vi "Machine_Etat_M1.vi"() -> ()   [LabVIEW 2017]
uses:
  Commande 1.ctl
  enum_tour.ctl
  <vilib>/Platform/TimedLoop/XDataNode/timing_clust.ctl
  <vilib>/Platform/TimedLoop/XDataNode/nitl_modes.ctl
  <vilib>/Platform/TimedLoop/XDataNode/wakeup.ctl
  <vilib>/myRIO/Instrument Drivers/Onboard IO/DIO/typedefs/DIO Reference.ctl
  <vilib>/myRIO/Common/Instrument Driver Framework/Utilities/typedefs/myRIO Generic Hardware Reference.ctl
  <vilib>/myRIO/Common/Instrument Driver Framework/Utilities/typedefs/Hardware Version Enum.ctl
  <vilib>/myRIO/Common/Instrument Driver Framework/Utilities/typedefs/myRIO v1.0 Reference.ctl
  <vilib>/myRIO/Common/Instrument Driver Framework/Utilities/typedefs/Generic FPGA Reference.ctl
  <vilib>/myRIO/Common/Instrument Driver Framework/myRIO v1.0/DIO/typedefs/DIO Channels List.ctl
  <vilib>/myRIO/Common/Instrument Driver Framework/myRIO v1.0/DIO/typedefs/DIO Channels Enum.ctl
  <vilib>/userdefined/High Color/nirio_resource_hc.ctl
  enum_bras.ctl
  <vilib>/myRIO/Common/Instrument Driver Framework/Utilities/vis/Is FPGA Ref Available.vi
  <vilib>/myRIO/Common/Instrument Driver Framework/myRIO v1.0/DIO/vis/myRIO v1.1 Open DIO.vi
  <vilib>/myRIO/Instrument Drivers/Onboard IO/DIO/vis/Write.vi
  <vilib>/myRIO/Common/Instrument Driver Framework/Utilities/vis/Validate Channels.vi
  <vilib>/myRIO/Common/Instrument Driver Framework/myRIO v1.0/DIO/vis/myRIO v1.0 Reserve DIO.vi
  <vilib>/myRIO/Common/Instrument Driver Framework/myRIO v1.0/Resource Manager/vis/myRIO v1.0 Reserve Channel List.vi
  <vilib>/myRIO/Common/Instrument Driver Framework/myRIO v1.0/DIO/vis/myRIO v1.0 Build MUX Configuration DIO.vi
  <vilib>/myRIO/Common/Instrument Driver Framework/myRIO v1.0/Resource Manager/vis/myRIO v1.0 Reserve Channel.vi
  <vilib>/myRIO/Common/Instrument Driver Framework/myRIO v1.0/Resource Manager/vis/myRIO v1.0 Unreserve Channel.vi
  <vilib>/myRIO/Common/Instrument Driver Framework/myRIO v1.0/Resource Manager/vis/myRIO v1.0 Create Configuration List.vi
  <vilib>/myRIO/Common/Instrument Driver Framework/myRIO v1.0/Resource Manager/vis/myRIO v1.0 Build Mutex Name.vi
  <vilib>/Utility/VariantDataType/GetNumericInfo.vi
  <vilib>/Utility/error.llb/Error Cluster From Error Code.vi
  <vilib>/myRIO/Common/Instrument Driver Framework/myRIO v1.0/myRIO v1.1 Open.vi
  <vilib>/myRIO/Common/Instrument Driver Framework/Utilities/vis/IO Manager.vi
  <vilib>/myRIO/Common/Instrument Driver Framework/Utilities/vis/Configuration Manager.vi
  <vilib>/myRIO/Common/Instrument Driver Framework/myRIO v1.0/Resource Manager/vis/myRIO v1.0 Configure IO.vi
  <vilib>/myRIO/Common/Instrument Driver Framework/myRIO v1.0/myRIO v1.0 Close.vi
  <vilib>/myRIO/Common/Instrument Driver Framework/myRIO v1.0/DIO/vis/myRIO v1.0 Write DIO.vi
  <vilib>/platform/TimedLoop/XDataNode/XDataNode.xnode
  <vilib>/myRIO/Express VI/Onboard Devices/LED/LED Express VI.xnode
  <vilib>/myRIO/Instrument Drivers/Onboard IO/DIO/vis/myRIO DIO Open.xnode
  <vilib>/Platform/TimedLoop/XDataNode/XDNodeRunTimeDep.lvlib
  <vilib>/myRIO/Instrument Drivers/Onboard IO/DIO/DIO.lvlib
panel:
  out "error out":errorcluster
  out "Vert : dévi à droite 2":bool
  out "Graphe déroulant 2":u32(graph)
  out "x > y ? 2":bool[](array[boolean])
  out "Cluster 3":T1
  out "4 LED droite 2":bool[](array[boolean])
  out "4 LED gauche 2":bool[](array[boolean])
  out "droite 2":u32
  out "gauche 2":u32
  out "Énum 2":T2
  out "seuil":u32
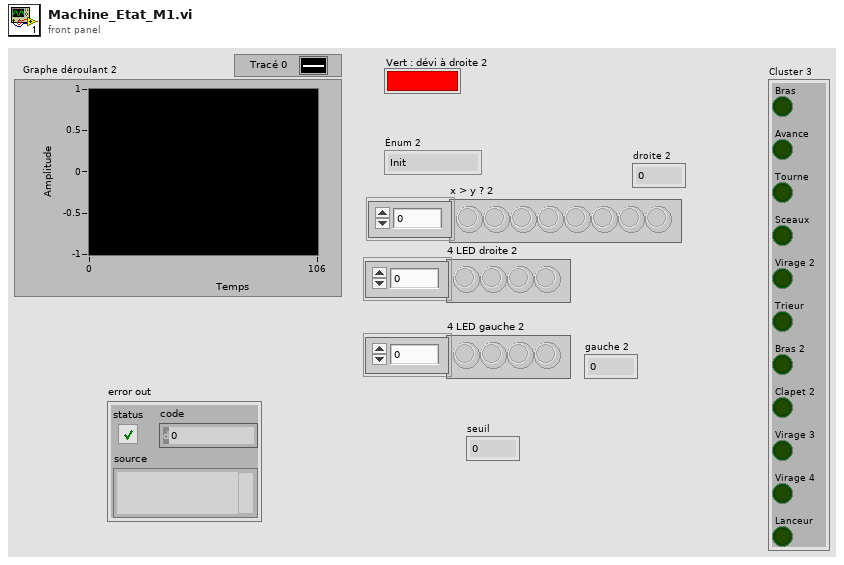
[diagram p1: front panel]
types:
  T1 = typedef "Voyant machine d'état.ctl" = cluster{"Bras":bool, "Avance":bool, "Tourne":bool, "Sceaux":bool, "Virage 2":bool, "Trieur":bool, "Bras 2":bool, "Clapet 2":bool, "Virage 3":bool, "Virage 4":bool, "Lanceur":bool}
  T2 = typedef "Commande 1.ctl" = enum16{"Init", "Bras", "Clapet 1", "Monter_bras", "Virage 1", "Sceaux 0", "Sceaux 1", "Sceaux 2", "Sceaux 3", "Sceaux 4", "Virage 2", "Recule", "Trieur", "Bras 2", "Intersection", "Clapet 2", "Virage 3", "Virage 4", "Avance", "Lanceur", "End", "Monter_bras1", "Monter_bras2", "Avance1", "Avance2", "Intersection1", "Avance3", "Demi_tour", "Virage 5", "Virage 6", "Intersection2", "Intersection3", "Intersection4"}
  T3 = typedef "enum_tour.ctl" = enum16{"Tour1", "Tour2", "Tour3"}
  T4 = typedef "XDNodeRunTimeDep.lvlib/timing_clust.ctl" = cluster{"Expected End [f-1]":u64, "Actual End [f-1]":u64, "Finished Late? [f-1]":bool, "Expected End [i-1]":u64, "Actual End [i-1]":u64, "Finished Late? [i-1]":bool, "Expected Start [i]":u64, "Actual Start [i]":u64, "Expected Start [f]":u64, "Actual Start [f]":u64, "Source Name":string, "Structure Name":string, "Period":i64, "Deadline":i64, "Offset":i64, "Start":i64, "Priority":i32, "Timeout":i32, "Mode":T5, "Wakeup Reason":T6, "Error":errorcluster, "Source Type":string, "Secondary Source Type":string, "Global End Time":u64, "Global Start Time":u64, "Frame Duration":u64, "Iteration Duration":u64, "Assigned CPU":i32, "I/O Scan Engine Mode":u32}
  T5 = typedef "XDNodeRunTimeDep.lvlib/nitl_modes.ctl" = enum32{"No Change", "Process missed periods, maintain original phase", "Discard missed periods, maintain original phase", "Process missed periods, ignore original phase", "Discard missed periods, ignore original phase"}
  T6 = typedef "XDNodeRunTimeDep.lvlib/wakeup.ctl" = enum32{"Normal", "Aborted", "Asynchronous wakeup", "Timing source error", "Timed loop error", "Timeout"}
  T7 = typedef "enum_bras.ctl" = enum16{"Depart Bras", "Clapet Bras", "Inactif Bras", "Seaux Bras"}
  T8 = typedef "DIO.lvlib/DIO Reference.ctl" = cluster{"myRIO Reference":T9, "DIO Channels List":T13}
  T9 = typedef "myRIO Generic Hardware Reference.ctl" = cluster{"myRIO Model":T10, "myRIO Hardware Reference":T11}
  T10 = typedef "Hardware Version Enum.ctl" = enum16{"Unknown", "myRIO-1900", "myRIO-1950", "roboRIO", "NI ELVIS RIO CM"}
  T11 = typedef "myRIO v1.0 Reference.ctl" = cluster{"Generic FPGA Reference":T12, "Allow multiple opens":bool}
  T12 = typedef "Generic FPGA Reference.ctl" = refnum<k20>
  T13 = typedef "DIO Channels List.ctl" = T14[]
  T14 = typedef "DIO Channels Enum.ctl" = enum16{"Not Connected", "C/DIO0", "C/DIO1", "C/DIO2", "C/DIO3", "C/DIO4", "C/DIO5", "C/DIO6", "C/DIO7", "A/DIO0", "A/DIO1", "A/DIO2", "A/DIO3", "A/DIO4", "A/DIO5", "A/DIO6", "A/DIO7", "A/DIO8", "A/DIO9", "A/DIO10", "A/DIO11", "A/DIO12", "A/DIO13", "A/DIO14", "A/DIO15", "B/DIO0", "B/DIO1", "B/DIO2", "B/DIO3", "B/DIO4", "B/DIO5", "B/DIO6", "B/DIO7", "B/DIO8", "B/DIO9", "B/DIO10", "B/DIO11", "B/DIO12", "B/DIO13", "B/DIO14", "B/DIO15", "LED0", "LED1", "LED2", "LED3", "Button0", "DIO/DIO0", "DIO/DIO1", "DIO/DIO2", "DIO/DIO3", "DIO/DIO4", "DIO/DIO5", "DIO/DIO6", "DIO/DIO7", "DIO/DIO8", "DIO/DIO9", "SPI/CS0", "SPI/CS1", "SPI/CS2", "SPI/CS3", "LED RADIO (Green)", "LED RADIO (Red)", "LED COMM (Green)", "LED COMM (Red)", "LED MODE (Green)", "LED MODE (Red)"}
  T15 = typedef "nirio_resource_hc.ctl" = tag
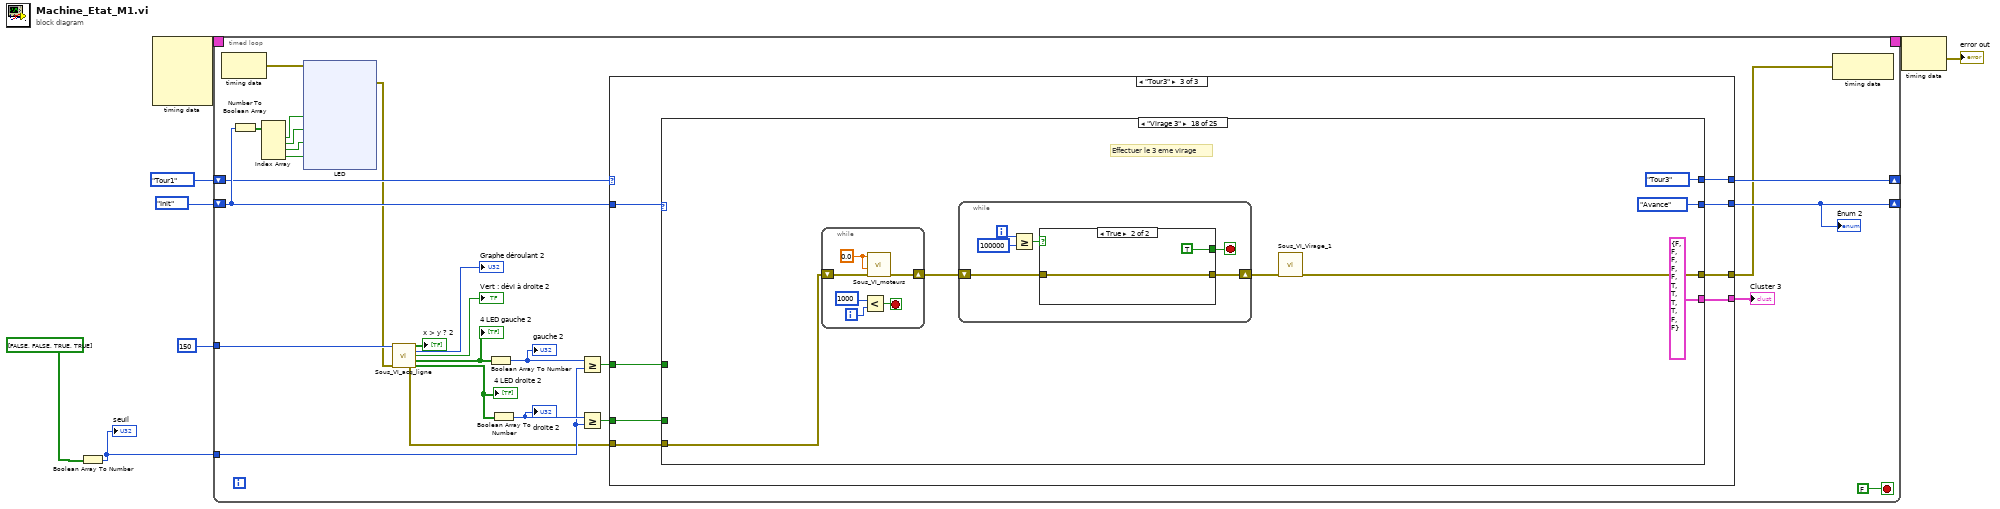
[diagram p0: block diagram]
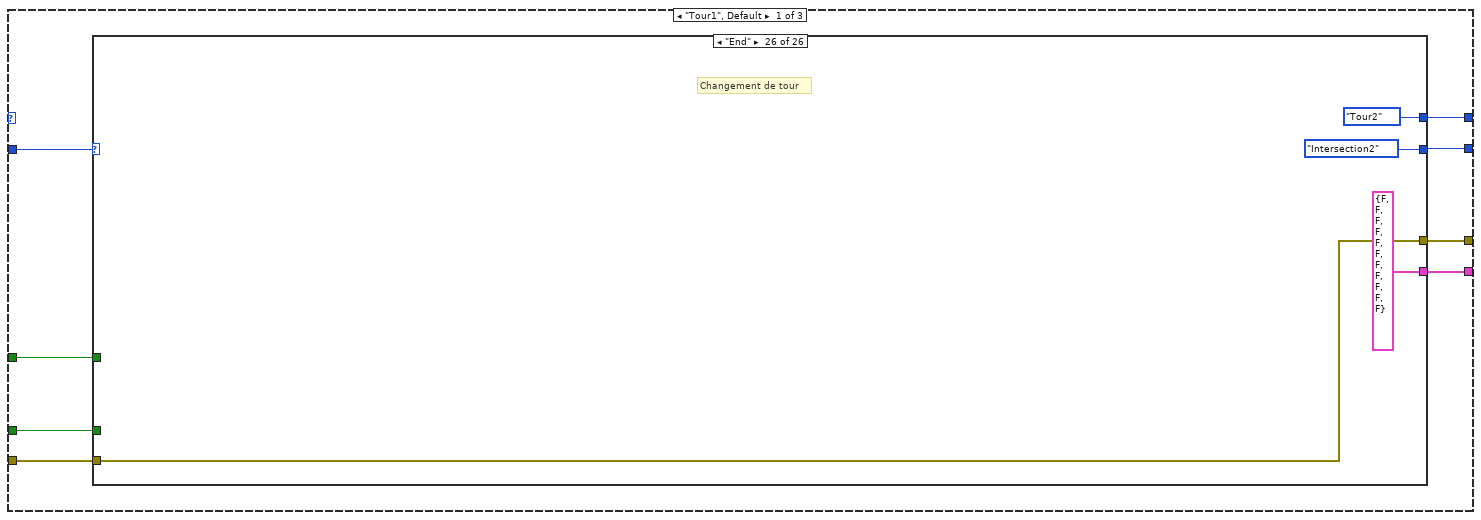
[diagram p2: hidden frame]
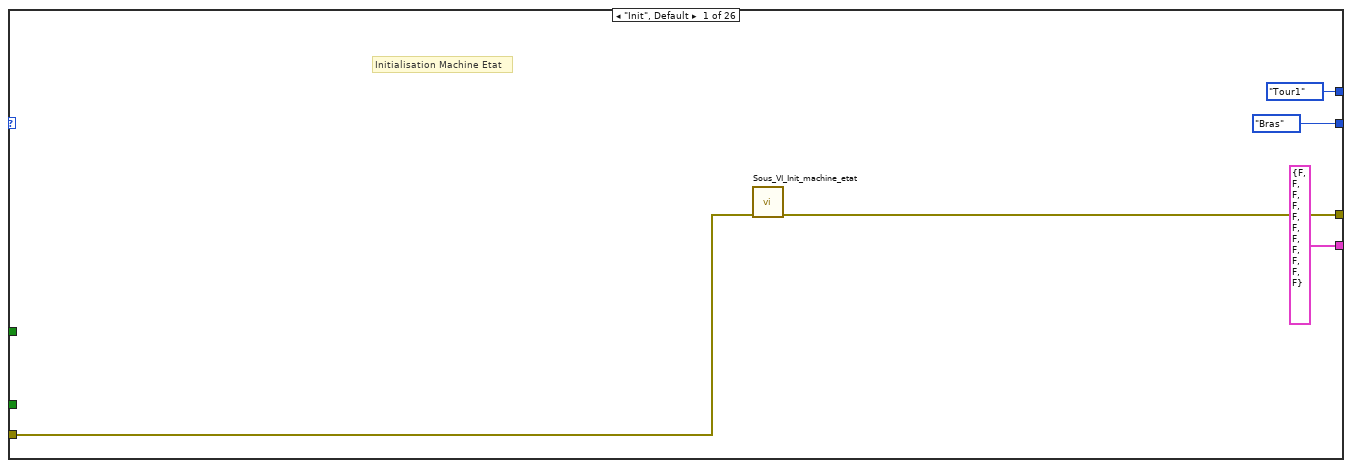
[diagram p3: hidden frame]
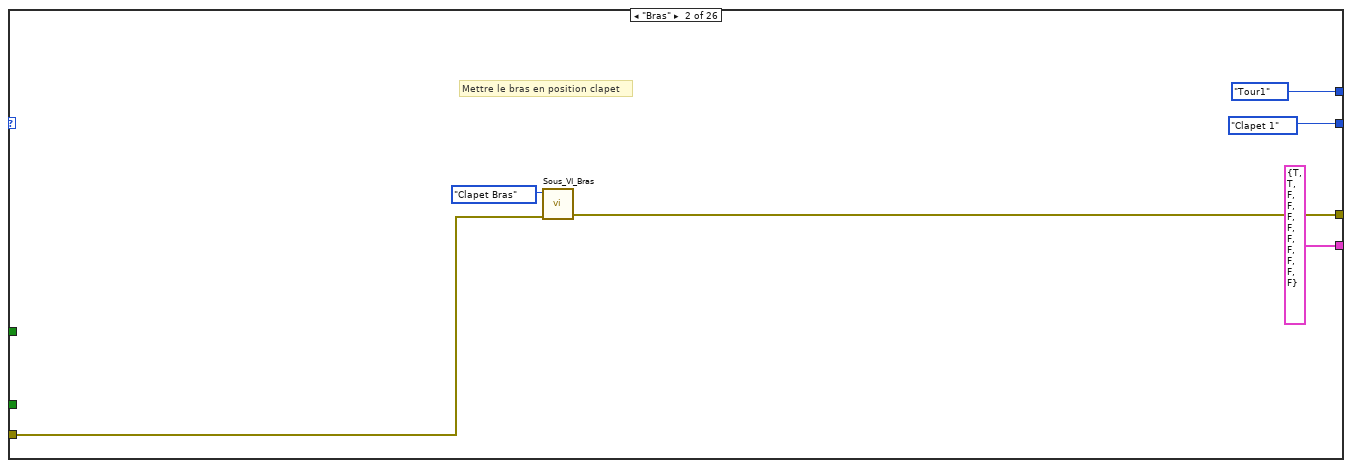
[diagram p4: hidden frame]
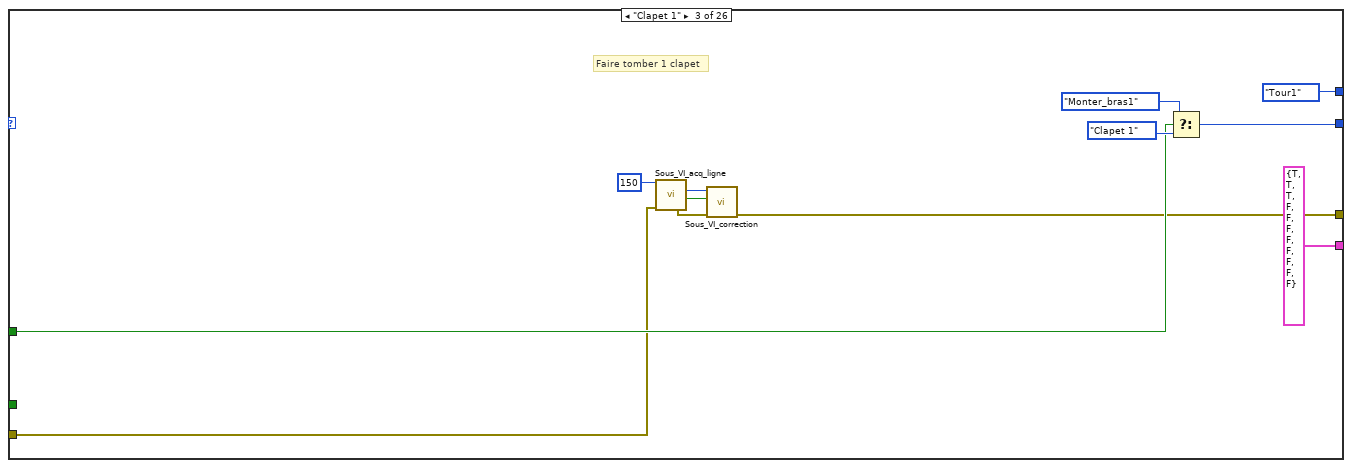
[diagram p5: hidden frame]
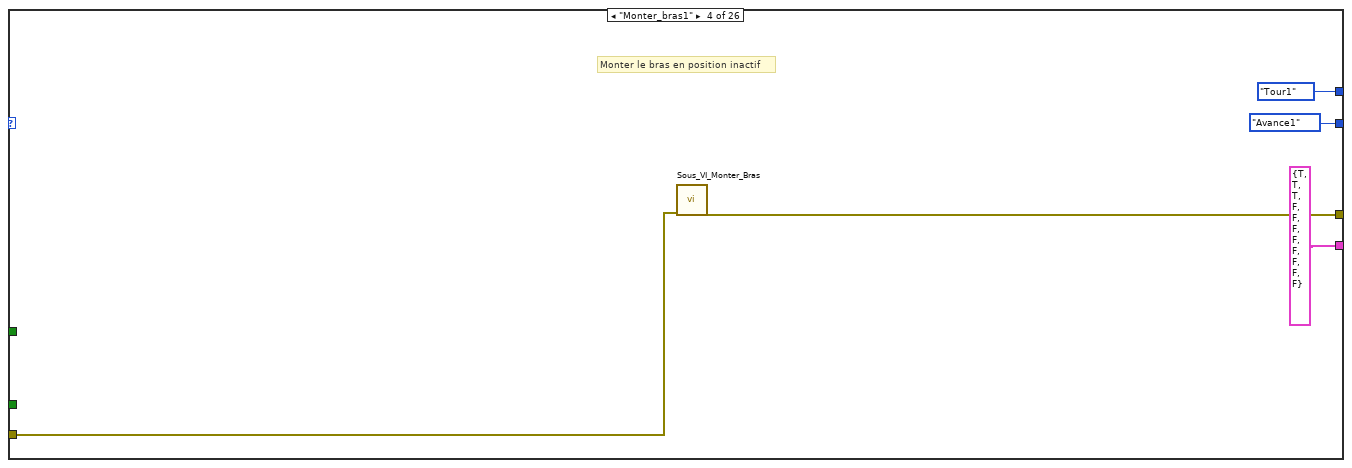
[diagram p6: hidden frame]
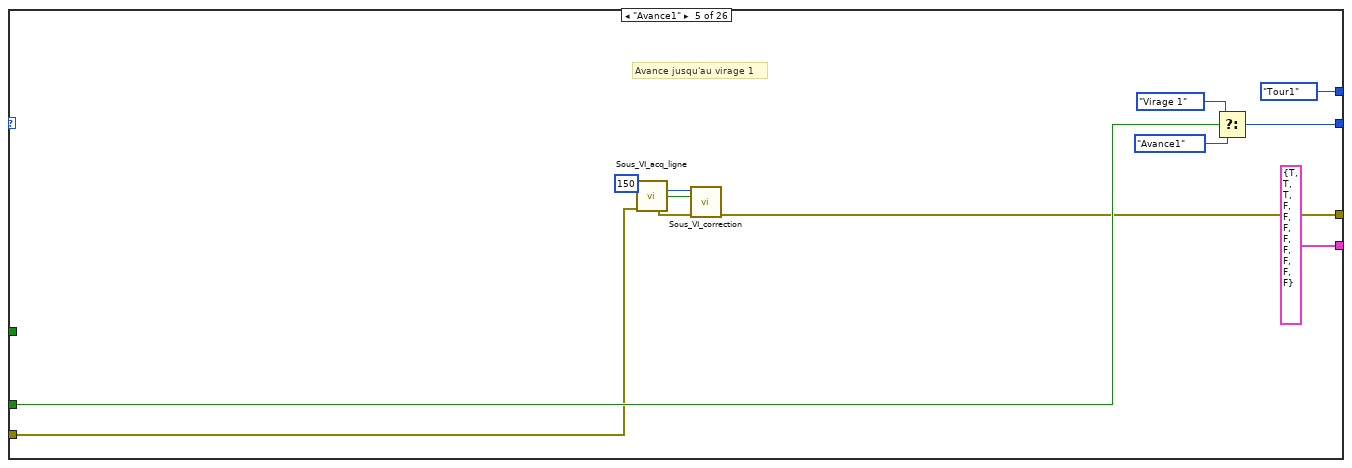
[diagram p7: hidden frame]
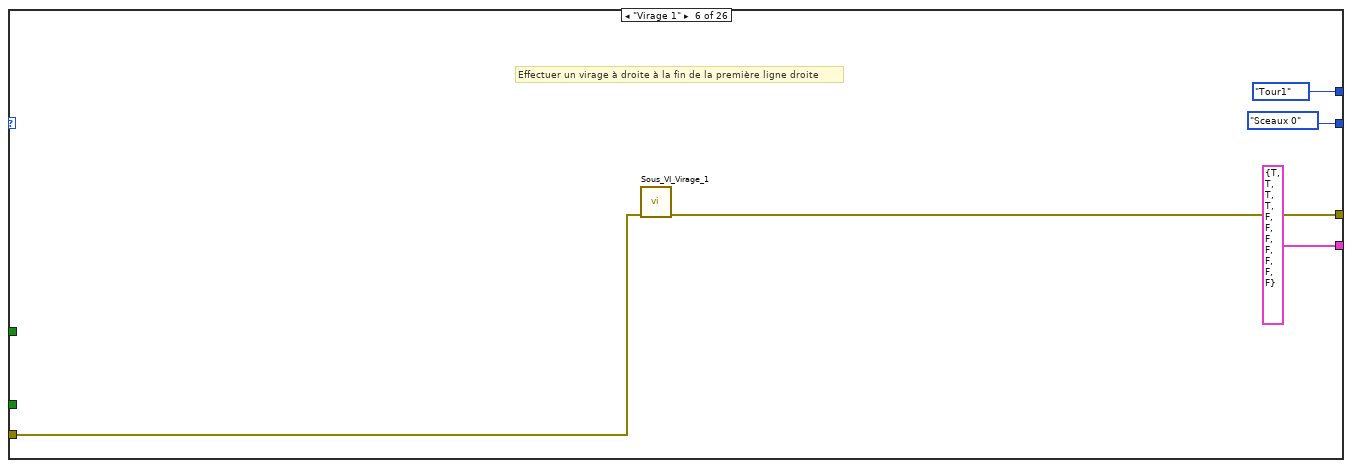
[diagram p8: hidden frame]
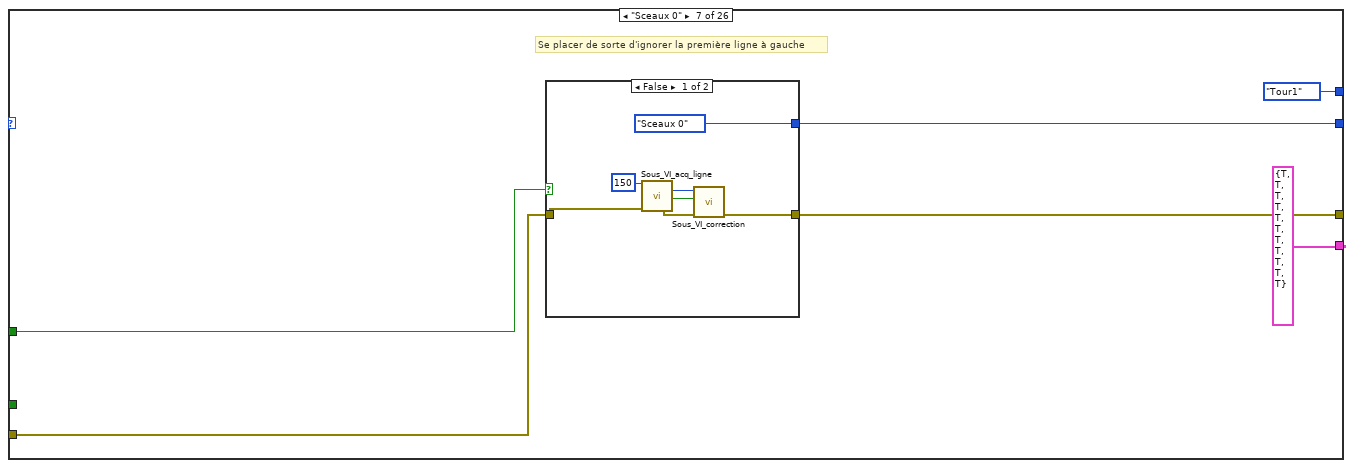
[diagram p9: hidden frame]
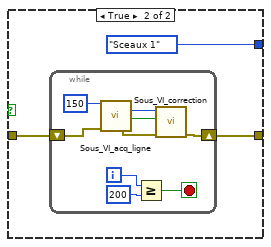
[diagram p10: hidden frame]
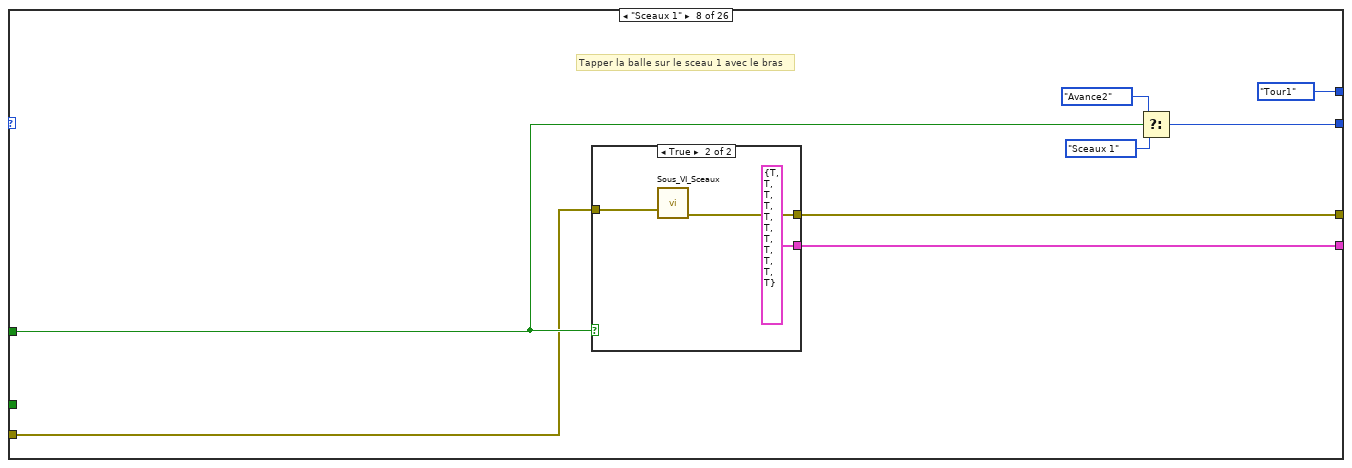
[diagram p11: hidden frame]
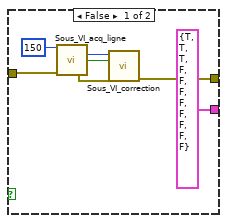
[diagram p12: hidden frame]
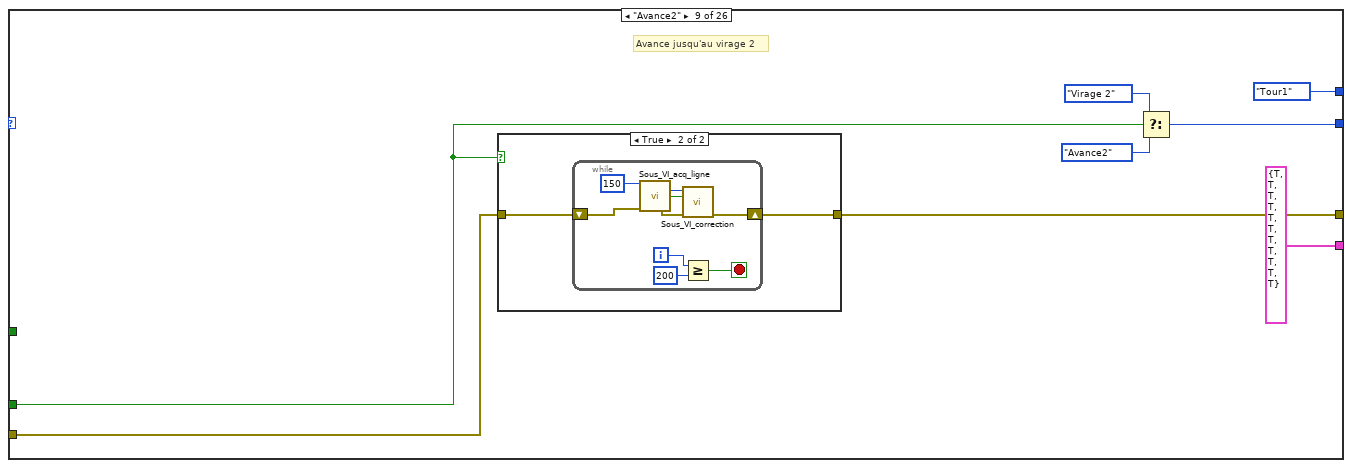
[diagram p13: hidden frame]
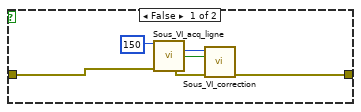
[diagram p14: hidden frame]
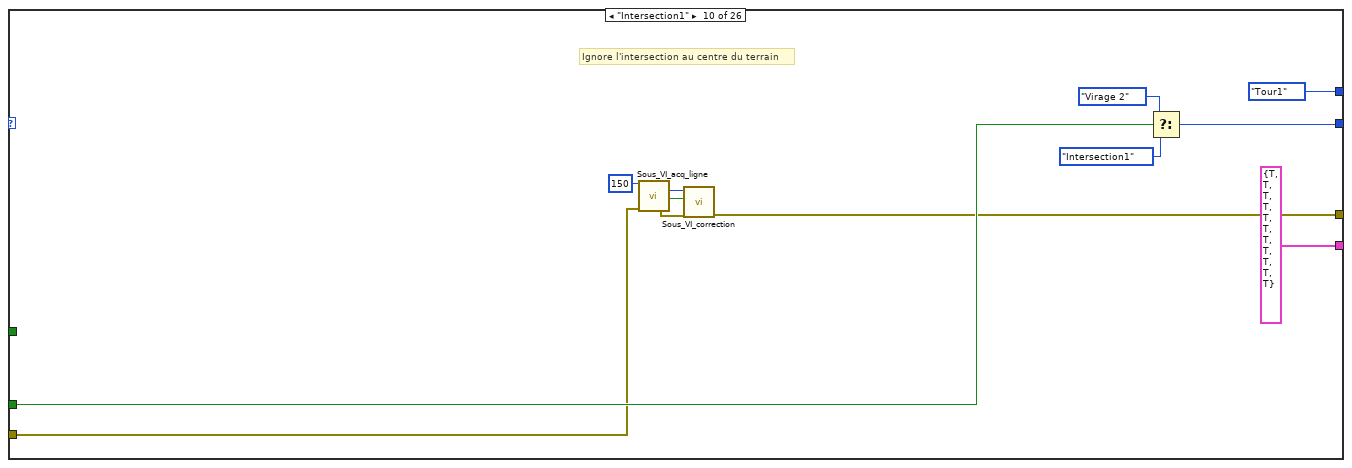
[diagram p15: hidden frame]
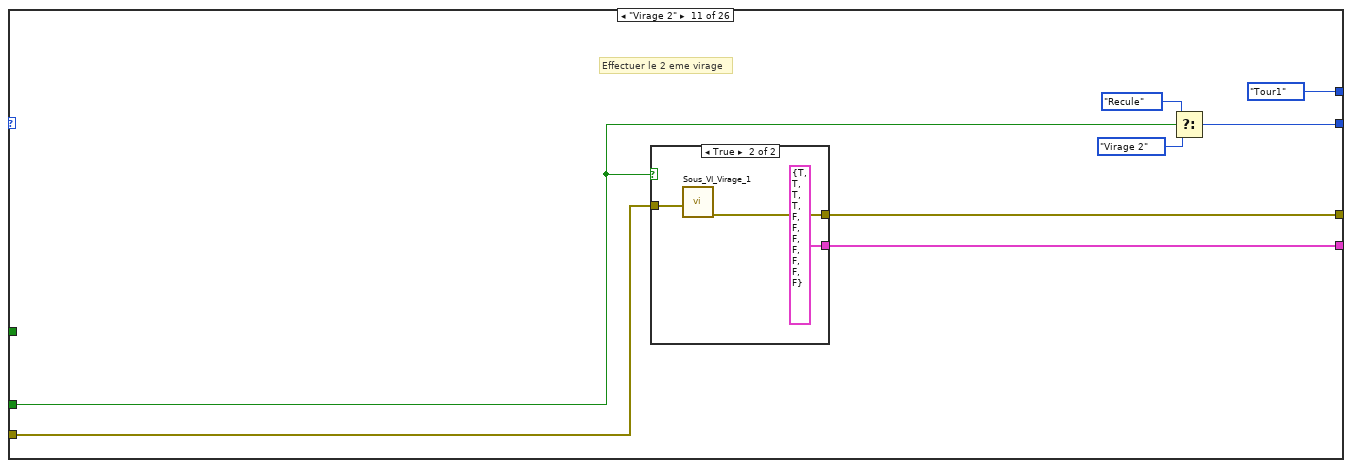
[diagram p16: hidden frame]
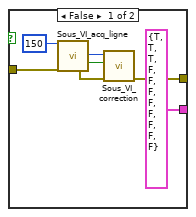
[diagram p17: hidden frame]
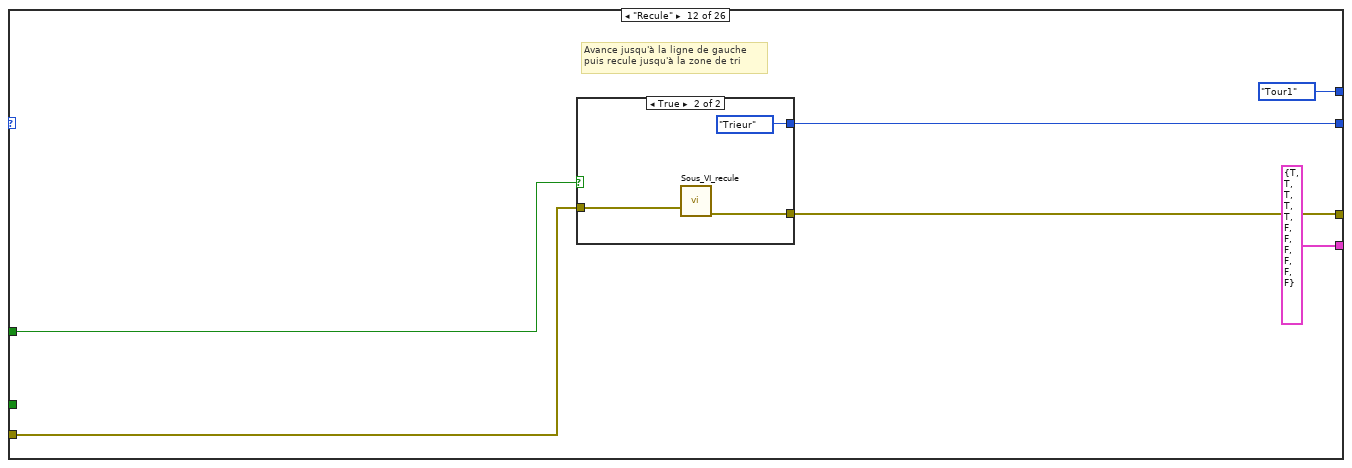
[diagram p18: hidden frame]
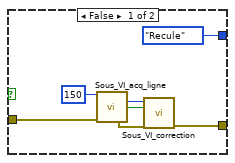
[diagram p19: hidden frame]
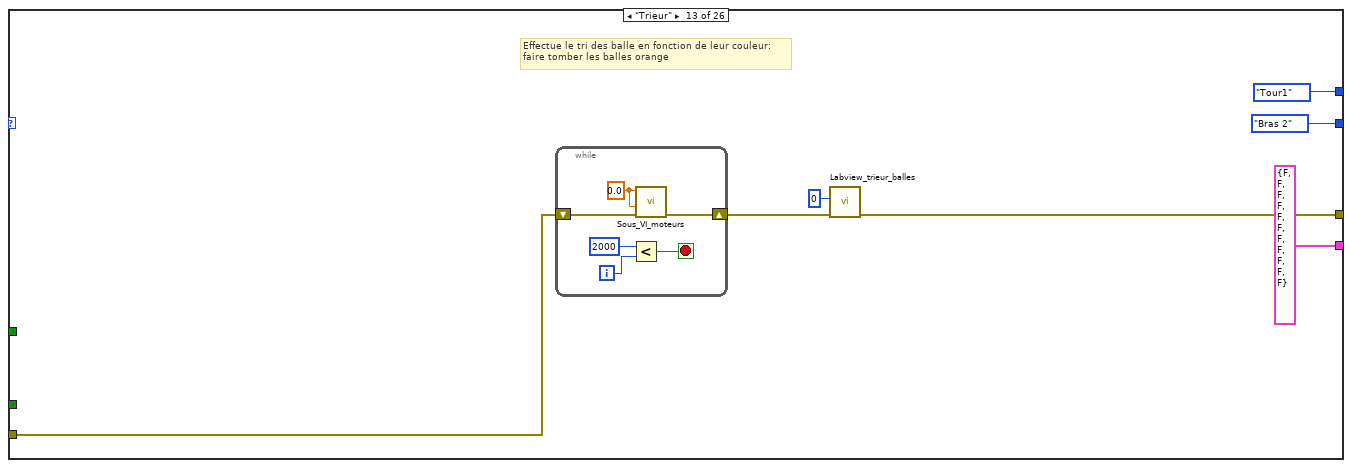
[diagram p20: hidden frame]
diagram:
  n1 = Boolean Array To Number(Boolean array=bool[] [FALSE, FALSE, TRUE, TRUE] ("x < y ? 2")) -> (number=w4:u32)
  "seuil" <- w4
  n2 = node-c288() -> (w7:T4)  [unwired: 4 in]
  n3 = timed-loop {
    tunnel: 150 ("value") -> [w29]
    shift-right: [w34] -> _
    shift-left: Commande_1."Init" -> [w21]
    tunnel: w4 -> [w23]
    timing: w7 -> [_]
    timing-out: [_] -> w6
    shift-right: [w13] -> _
    shift-left: enum_tour."Tour1" -> [w14]
    stop <- FALSE stop-if-true
    n4 = node-c288() -> (w12:errorcluster)  [unwired: 1 in]
    n5 = Number To Boolean Array(number=w21) -> (Boolean array=w20:bool[])
    n6 = Index Array(array=w20) -> (element #1=w19:bool, element #2=w18:bool, element #3=w17:bool, element #4=w16:bool)  [unwired: 4 in]
    n7 = xnode "LED"("LED0"=w19, "LED1"=w18, "LED2"=w17, "LED3"=w16, "error in (no error)"=w12) -> ("error out"=w11:errorcluster)
    n8 = call "Sous_VI_acq_ligne.vi"("Seuil"=w29, "error in (no error)"=w11) -> ("x > y ?"=→"x > y ? 2":bool[], "Décalage"=→"Graphe déroulant 2":u32, "G/D ?"=→"Vert : dévi à droite 2":bool, "4 LED gauches"=w26:bool[], "error out"=w10:errorcluster, "4 LED droite"=w25:bool[])  [unwired: 8 in]
    "4 LED droite 2" <- w25
    "4 LED gauche 2" <- w26
    n9 = Boolean Array To Number(Boolean array=w26) -> (number=w22:u32)
    "gauche 2" <- w22
    n10 = Boolean Array To Number(Boolean array=w25) -> (number=w24:u32)
    "droite 2" <- w24
    n11 = Greater Or Equal?(x=w22, y=w23) -> (x >= y?=w32:bool)
    n12 = Greater Or Equal?(x=w24, y=w23) -> (x >= y?=w33:bool)
    n13 = case shown="\"Tour3\"" w14 {
      tunnel: [w42 w348 w709] -> w34
      tunnel: w33 -> [w41 w344 w705]
      tunnel: w32 -> [w40 w345 w706]
      tunnel: [w39 w347 w708] -> w28
      tunnel: w21 -> [w38 w349 w704]
      tunnel: [w37 w346 w707] -> w13
      tunnel: w10 -> [w36 w343 w703]
      tunnel: [w35 w342 w702] -> w9
      frame "Tour1", Default {
        n14 = case shown="\"End\"" w38 {
          tunnel: [Commande_1."Bras" Commande_1."Clapet 1" w63 Commande_1."Avance1" w76 Commande_1."Sceaux 0" w93 w118 w135 w161 w172 w189 Commande_1."Bras 2" Commande_1."Clapet 2" w239 w250 Commande_1."Avance3" w267 Commande_1."Avance" w286 Commande_1."Lanceur" Commande_1."Demi_tour" Commande_1."Virage 5" w311 w326 Commande_1."Intersection2"] -> w42
          tunnel: w41 -> [_ _ _ _ w77 _ _ _ w133 w162 w171 _ _ _ w237 _ _ w266 _ w285 _ _ _ w310 w327 _]
          tunnel: [T1 {"Bras"=FALSE, "Avance"=FALSE, "Tourne"=FALSE, "Sceaux"=FALSE, "Virage 2"=FALSE, "Trieur"=FALSE, "Bras 2"=FALSE, "Clapet 2"=FALSE, "Virage 3"=FALSE, "Virage 4"=FALSE, "Lanceur"=FALSE} ("Cluster 2") T1 {"Bras"=TRUE, "Avance"=TRUE, "Tourne"=FALSE, "Sceaux"=FALSE, "Virage 2"=FALSE, "Trieur"=FALSE, "Bras 2"=FALSE, "Clapet 2"=FALSE, "Virage 3"=FALSE, "Virage 4"=FALSE, "Lanceur"=FALSE} ("Cluster 2") T1 {"Bras"=TRUE, "Avance"=TRUE, "Tourne"=TRUE, "Sceaux"=FALSE, "Virage 2"=FALSE, "Trieur"=FALSE, "Bras 2"=FALSE, "Clapet 2"=FALSE, "Virage 3"=FALSE, "Virage 4"=FALSE, "Lanceur"=FALSE} ("Cluster 2") T1 {"Bras"=TRUE, "Avance"=TRUE, "Tourne"=TRUE, "Sceaux"=FALSE, "Virage 2"=FALSE, "Trieur"=FALSE, "Bras 2"=FALSE, "Clapet 2"=FALSE, "Virage 3"=FALSE, "Virage 4"=FALSE, "Lanceur"=FALSE} ("Cluster 2") T1 {"Bras"=TRUE, "Avance"=TRUE, "Tourne"=TRUE, "Sceaux"=FALSE, "Virage 2"=FALSE, "Trieur"=FALSE, "Bras 2"=FALSE, "Clapet 2"=FALSE, "Virage 3"=FALSE, "Virage 4"=FALSE, "Lanceur"=FALSE} ("Cluster 2") T1 {"Bras"=TRUE, "Avance"=TRUE, "Tourne"=TRUE, "Sceaux"=TRUE, "Virage 2"=FALSE, "Trieur"=FALSE, "Bras 2"=FALSE, "Clapet 2"=FALSE, "Virage 3"=FALSE, "Virage 4"=FALSE, "Lanceur"=FALSE} ("Cluster 2") T1 {"Bras"=TRUE, "Avance"=TRUE, "Tourne"=TRUE, "Sceaux"=TRUE, "Virage 2"=TRUE, "Trieur"=TRUE, "Bras 2"=TRUE, "Clapet 2"=TRUE, "Virage 3"=TRUE, "Virage 4"=TRUE, "Lanceur"=TRUE} ("Cluster 2") w117 T1 {"Bras"=TRUE, "Avance"=TRUE, "Tourne"=TRUE, "Sceaux"=TRUE, "Virage 2"=TRUE, "Trieur"=TRUE, "Bras 2"=TRUE, "Clapet 2"=TRUE, "Virage 3"=TRUE, "Virage 4"=TRUE, "Lanceur"=TRUE} ("Cluster 2") T1 {"Bras"=TRUE, "Avance"=TRUE, "Tourne"=TRUE, "Sceaux"=TRUE, "Virage 2"=TRUE, "Trieur"=TRUE, "Bras 2"=TRUE, "Clapet 2"=TRUE, "Virage 3"=TRUE, "Virage 4"=TRUE, "Lanceur"=TRUE} ("Cluster 2") w175 T1 {"Bras"=TRUE, "Avance"=TRUE, "Tourne"=TRUE, "Sceaux"=TRUE, "Virage 2"=TRUE, "Trieur"=FALSE, "Bras 2"=FALSE, "Clapet 2"=FALSE, "Virage 3"=FALSE, "Virage 4"=FALSE, "Lanceur"=FALSE} ("Cluster 2") T1 {"Bras"=FALSE, "Avance"=FALSE, "Tourne"=FALSE, "Sceaux"=FALSE, "Virage 2"=FALSE, "Trieur"=FALSE, "Bras 2"=FALSE, "Clapet 2"=FALSE, "Virage 3"=FALSE, "Virage 4"=FALSE, "Lanceur"=FALSE} ("Cluster 2") T1 {"Bras"=FALSE, "Avance"=FALSE, "Tourne"=FALSE, "Sceaux"=FALSE, "Virage 2"=FALSE, "Trieur"=TRUE, "Bras 2"=FALSE, "Clapet 2"=FALSE, "Virage 3"=FALSE, "Virage 4"=FALSE, "Lanceur"=FALSE} ("Cluster 2") T1 {"Bras"=FALSE, "Avance"=FALSE, "Tourne"=FALSE, "Sceaux"=FALSE, "Virage 2"=FALSE, "Trieur"=TRUE, "Bras 2"=TRUE, "Clapet 2"=FALSE, "Virage 3"=FALSE, "Virage 4"=FALSE, "Lanceur"=FALSE} ("Cluster 2") T1 {"Bras"=FALSE, "Avance"=FALSE, "Tourne"=FALSE, "Sceaux"=FALSE, "Virage 2"=FALSE, "Trieur"=TRUE, "Bras 2"=TRUE, "Clapet 2"=FALSE, "Virage 3"=FALSE, "Virage 4"=FALSE, "Lanceur"=FALSE} ("Cluster 2") T1 {"Bras"=TRUE, "Avance"=TRUE, "Tourne"=TRUE, "Sceaux"=FALSE, "Virage 2"=FALSE, "Trieur"=FALSE, "Bras 2"=FALSE, "Clapet 2"=FALSE, "Virage 3"=FALSE, "Virage 4"=FALSE, "Lanceur"=FALSE} ("Cluster 2") T1 {"Bras"=TRUE, "Avance"=TRUE, "Tourne"=TRUE, "Sceaux"=TRUE, "Virage 2"=TRUE, "Trieur"=TRUE, "Bras 2"=TRUE, "Clapet 2"=TRUE, "Virage 3"=TRUE, "Virage 4"=TRUE, "Lanceur"=TRUE} ("Cluster 2") T1 {"Bras"=FALSE, "Avance"=FALSE, "Tourne"=FALSE, "Sceaux"=FALSE, "Virage 2"=FALSE, "Trieur"=TRUE, "Bras 2"=TRUE, "Clapet 2"=TRUE, "Virage 3"=TRUE, "Virage 4"=FALSE, "Lanceur"=FALSE} ("Cluster 2") T1 {"Bras"=FALSE, "Avance"=FALSE, "Tourne"=FALSE, "Sceaux"=FALSE, "Virage 2"=FALSE, "Trieur"=FALSE, "Bras 2"=TRUE, "Clapet 2"=TRUE, "Virage 3"=TRUE, "Virage 4"=TRUE, "Lanceur"=FALSE} ("Cluster 2") T1 {"Bras"=FALSE, "Avance"=FALSE, "Tourne"=FALSE, "Sceaux"=FALSE, "Virage 2"=FALSE, "Trieur"=TRUE, "Bras 2"=TRUE, "Clapet 2"=TRUE, "Virage 3"=TRUE, "Virage 4"=TRUE, "Lanceur"=FALSE} ("Cluster 2") T1 {"Bras"=FALSE, "Avance"=FALSE, "Tourne"=FALSE, "Sceaux"=FALSE, "Virage 2"=FALSE, "Trieur"=FALSE, "Bras 2"=TRUE, "Clapet 2"=TRUE, "Virage 3"=TRUE, "Virage 4"=TRUE, "Lanceur"=TRUE} ("Cluster 2") T1 {"Bras"=FALSE, "Avance"=FALSE, "Tourne"=FALSE, "Sceaux"=FALSE, "Virage 2"=FALSE, "Trieur"=TRUE, "Bras 2"=TRUE, "Clapet 2"=TRUE, "Virage 3"=TRUE, "Virage 4"=TRUE, "Lanceur"=FALSE} ("Cluster 2") T1 {"Bras"=FALSE, "Avance"=FALSE, "Tourne"=FALSE, "Sceaux"=FALSE, "Virage 2"=FALSE, "Trieur"=TRUE, "Bras 2"=TRUE, "Clapet 2"=TRUE, "Virage 3"=TRUE, "Virage 4"=TRUE, "Lanceur"=FALSE} ("Cluster 2") T1 {"Bras"=FALSE, "Avance"=FALSE, "Tourne"=FALSE, "Sceaux"=FALSE, "Virage 2"=FALSE, "Trieur"=TRUE, "Bras 2"=TRUE, "Clapet 2"=TRUE, "Virage 3"=TRUE, "Virage 4"=TRUE, "Lanceur"=FALSE} ("Cluster 2") T1 {"Bras"=FALSE, "Avance"=FALSE, "Tourne"=FALSE, "Sceaux"=FALSE, "Virage 2"=FALSE, "Trieur"=FALSE, "Bras 2"=FALSE, "Clapet 2"=FALSE, "Virage 3"=FALSE, "Virage 4"=FALSE, "Lanceur"=FALSE} ("Cluster 2")] -> w39
          tunnel: w40 -> [_ _ w59 _ _ _ w92 w116 _ _ _ w190 _ _ _ w248 _ _ _ _ _ _ _ _ _ _]
          tunnel: [enum_tour."Tour1" enum_tour."Tour1" enum_tour."Tour1" enum_tour."Tour1" enum_tour."Tour1" enum_tour."Tour1" enum_tour."Tour1" enum_tour."Tour1" enum_tour."Tour1" enum_tour."Tour1" enum_tour."Tour1" enum_tour."Tour1" enum_tour."Tour1" enum_tour."Tour1" enum_tour."Tour1" enum_tour."Tour1" enum_tour."Tour1" enum_tour."Tour1" enum_tour."Tour1" enum_tour."Tour1" enum_tour."Tour1" enum_tour."Tour1" enum_tour."Tour1" enum_tour."Tour1" enum_tour."Tour1" enum_tour."Tour2"] -> w37
          tunnel: w36 -> [w44 w49 w55 w66 w74 w84 w89 w113 w132 w157 w168 w186 w202 w215 w232 w244 w256 w261 w273 w278 w290 w296 w301 w306 w322 w338]
          tunnel: [w43 w48 w54 w67 w71 w83 w88 w114 w131 w156 w169 w187 w203 w216 w233 w245 w257 w262 w274 w279 w291 w295 w302 w307 w323 w338] -> w35
          frame "Init", Default {
            # "Initialisation Machine Etat"
            n15 = call "Sous_VI_Init_machine_etat.vi"("error in (no error)"=w44) -> ("error out"=w43:errorcluster)  [unwired: 10 in]
          }
          frame "Bras" {
            # "Mettre le bras en position clapet"
            n16 = call "Sous_VI_Bras.vi"("error in (no error)"=w49, "Enum bras"=enum_bras."Clapet Bras") -> ("error out"=w48:errorcluster)  [unwired: 9 in]
          }
          frame "Clapet 1" {
            # "Faire tomber 1 clapet"
            n17 = call "Sous_VI_acq_ligne.vi"("Seuil"=150, "error in (no error)"=w55) -> ("Décalage"=w61:u32, "G/D ?"=w57:bool, "error out"=w56:errorcluster)  [unwired: 8 in, 3 out]
            n18 = call "Sous_VI_correction.vi"("error in (no error)"=w56, "G/D ?"=w57, "Décalage"=w61) -> ("error out"=w54:errorcluster)  [unwired: 8 in]
            n19 = Select(t=Commande_1."Monter_bras1", s=w59, f=Commande_1."Clapet 1") -> (s? t:f=w63:T2)
          }
          frame "Monter_bras1" {
            # "Monter le bras en position inactif"
            n20 = call "Sous_VI_Monter_Bras.vi"("error in (no error)"=w66) -> ("error out"=w67:errorcluster)  [unwired: 10 in]
          }
          frame "Avance1" {
            # "Avance jusqu'au virage 1"
            n21 = call "Sous_VI_acq_ligne.vi"("Seuil"=150, "error in (no error)"=w74) -> ("Décalage"=w79:u32, "G/D ?"=w72:bool, "error out"=w73:errorcluster)  [unwired: 8 in, 3 out]
            n22 = call "Sous_VI_correction.vi"("error in (no error)"=w73, "G/D ?"=w72, "Décalage"=w79) -> ("error out"=w71:errorcluster)  [unwired: 8 in]
            n23 = Select(t=Commande_1."Virage 1", s=w77, f=Commande_1."Avance1") -> (s? t:f=w76:T2)
          }
          frame "Virage 1" {
            # "Effectuer un virage à droite à la fin de la première ligne droite"
            n24 = call "Sous_VI_Virage_1.vi"("error in (no error)"=w84) -> ("error out"=w83:errorcluster)  [unwired: 10 in]
          }
          frame "Sceaux 0" {
            # "Se placer de sorte d'ignorer la première ligne à gauche"
            n25 = case shown="False" w92 {
              tunnel: [Commande_1."Sceaux 0" Commande_1."Sceaux 1"] -> w93
              tunnel: w89 -> [w95 w102]
              tunnel: [w94 w101] -> w88
              frame False {
                n26 = call "Sous_VI_acq_ligne.vi"("Seuil"=150, "error in (no error)"=w95) -> ("Décalage"=w99:u32, "G/D ?"=w96:bool, "error out"=w97:errorcluster)  [unwired: 8 in, 3 out]
                n27 = call "Sous_VI_correction.vi"("error in (no error)"=w97, "G/D ?"=w96, "Décalage"=w99) -> ("error out"=w94:errorcluster)  [unwired: 8 in]
              }
              frame True {
                n28 = while {
                  shift-right: [w104] -> w101
                  shift-left: w102 -> [w105]
                  i -> [w112]
                  stop <- w108 stop-if-true
                  n29 = call "Sous_VI_acq_ligne.vi"("Seuil"=150, "error in (no error)"=w105) -> ("Décalage"=w109:u32, "G/D ?"=w106:bool, "error out"=w107:errorcluster)  [unwired: 8 in, 3 out]
                  n30 = Greater Or Equal?(x=w112, y=200) -> (x >= y?=w108:bool)
                  n31 = call "Sous_VI_correction.vi"("error in (no error)"=w107, "G/D ?"=w106, "Décalage"=w109) -> ("error out"=w104:errorcluster)  [unwired: 8 in]
                }
              }
            }
          }
          frame "Sceaux 1" {
            # "Tapper la balle sur le sceau 1 avec le bras"
            n32 = case shown="True" w116 {
              tunnel: [T1 {"Bras"=TRUE, "Avance"=TRUE, "Tourne"=TRUE, "Sceaux"=FALSE, "Virage 2"=FALSE, "Trieur"=FALSE, "Bras 2"=FALSE, "Clapet 2"=FALSE, "Virage 3"=FALSE, "Virage 4"=FALSE, "Lanceur"=FALSE} ("Cluster 2") T1 {"Bras"=TRUE, "Avance"=TRUE, "Tourne"=TRUE, "Sceaux"=TRUE, "Virage 2"=TRUE, "Trieur"=TRUE, "Bras 2"=TRUE, "Clapet 2"=TRUE, "Virage 3"=TRUE, "Virage 4"=TRUE, "Lanceur"=TRUE} ("Cluster 2")] -> w117
              tunnel: [w122 w129] -> w114
              tunnel: w113 -> [w121 w128]
              frame False {
                n33 = call "Sous_VI_acq_ligne.vi"("Seuil"=150, "error in (no error)"=w121) -> ("Décalage"=w126:u32, "G/D ?"=w123:bool, "error out"=w124:errorcluster)  [unwired: 8 in, 3 out]
                n34 = call "Sous_VI_correction.vi"("error in (no error)"=w124, "G/D ?"=w123, "Décalage"=w126) -> ("error out"=w122:errorcluster)  [unwired: 8 in]
              }
              frame True {
                n35 = call "Sous_VI_Sceaux.vi"("error in (no error)"=w128) -> ("error out"=w129:errorcluster)  [unwired: 10 in]
              }
            }
            n36 = Select(t=Commande_1."Avance2", s=w116, f=Commande_1."Sceaux 1") -> (s? t:f=w118:T2)
          }
          frame "Avance2" {
            # "Avance jusqu'au virage 2"
            n37 = case shown="True" w133 {
              tunnel: w132 -> [w140 w146]
              tunnel: [w139 w145] -> w131
              frame False {
                n38 = call "Sous_VI_acq_ligne.vi"("Seuil"=150, "error in (no error)"=w140) -> ("Décalage"=w143:u32, "G/D ?"=w141:bool, "error out"=w142:errorcluster)  [unwired: 8 in, 3 out]
                n39 = call "Sous_VI_correction.vi"("error in (no error)"=w142, "G/D ?"=w141, "Décalage"=w143) -> ("error out"=w139:errorcluster)  [unwired: 8 in]
              }
              frame True {
                n40 = while {
                  shift-right: [w147] -> w145
                  shift-left: w146 -> [w148]
                  i -> [w155]
                  stop <- w151 stop-if-true
                  n41 = call "Sous_VI_acq_ligne.vi"("Seuil"=150, "error in (no error)"=w148) -> ("Décalage"=w152:u32, "G/D ?"=w149:bool, "error out"=w150:errorcluster)  [unwired: 8 in, 3 out]
                  n42 = call "Sous_VI_correction.vi"("error in (no error)"=w150, "G/D ?"=w149, "Décalage"=w152) -> ("error out"=w147:errorcluster)  [unwired: 8 in]
                  n43 = Greater Or Equal?(x=w155, y=200) -> (x >= y?=w151:bool)
                }
              }
            }
            n44 = Select(t=Commande_1."Virage 2", s=w133, f=Commande_1."Avance2") -> (s? t:f=w135:T2)
          }
          frame "Intersection1" {
            # "Ignore l'intersection au centre du terrain"
            n45 = call "Sous_VI_acq_ligne.vi"("Seuil"=150, "error in (no error)"=w157) -> ("Décalage"=w165:u32, "G/D ?"=w158:bool, "error out"=w159:errorcluster)  [unwired: 8 in, 3 out]
            n46 = call "Sous_VI_correction.vi"("error in (no error)"=w159, "G/D ?"=w158, "Décalage"=w165) -> ("error out"=w156:errorcluster)  [unwired: 8 in]
            n47 = Select(t=Commande_1."Virage 2", s=w162, f=Commande_1."Intersection1") -> (s? t:f=w161:T2)
          }
          frame "Virage 2" {
            # "Effectuer le 2 eme virage"
            n48 = case shown="True" w171 {
              tunnel: [T1 {"Bras"=TRUE, "Avance"=TRUE, "Tourne"=TRUE, "Sceaux"=FALSE, "Virage 2"=FALSE, "Trieur"=FALSE, "Bras 2"=FALSE, "Clapet 2"=FALSE, "Virage 3"=FALSE, "Virage 4"=FALSE, "Lanceur"=FALSE} ("Cluster 2") T1 {"Bras"=TRUE, "Avance"=TRUE, "Tourne"=TRUE, "Sceaux"=TRUE, "Virage 2"=FALSE, "Trieur"=FALSE, "Bras 2"=FALSE, "Clapet 2"=FALSE, "Virage 3"=FALSE, "Virage 4"=FALSE, "Lanceur"=FALSE} ("Cluster 2")] -> w175
              tunnel: [w177 w184] -> w169
              tunnel: w168 -> [w176 w183]
              frame False {
                n49 = call "Sous_VI_acq_ligne.vi"("Seuil"=150, "error in (no error)"=w176) -> ("Décalage"=w181:u32, "G/D ?"=w179:bool, "error out"=w178:errorcluster)  [unwired: 8 in, 3 out]
                n50 = call "Sous_VI_correction.vi"("error in (no error)"=w178, "G/D ?"=w179, "Décalage"=w181) -> ("error out"=w177:errorcluster)  [unwired: 8 in]
              }
              frame True {
                n51 = call "Sous_VI_Virage_1.vi"("error in (no error)"=w183) -> ("error out"=w184:errorcluster)  [unwired: 10 in]
              }
            }
            n52 = Select(t=Commande_1."Recule", s=w171, f=Commande_1."Virage 2") -> (s? t:f=w172:T2)
          }
          frame "Recule" {
            # "Avance jusqu'à la ligne de gauche \npuis recule jusqu'à la zone de tri"
            n53 = case shown="True" w190 {
              tunnel: [Commande_1."Recule" Commande_1."Trieur"] -> w189
              tunnel: [w193 w200] -> w187
              tunnel: w186 -> [w192 w199]
              frame False {
                n54 = call "Sous_VI_acq_ligne.vi"("Seuil"=150, "error in (no error)"=w192) -> ("Décalage"=w196:u32, "G/D ?"=w195:bool, "error out"=w194:errorcluster)  [unwired: 8 in, 3 out]
                n55 = call "Sous_VI_correction.vi"("error in (no error)"=w194, "G/D ?"=w195, "Décalage"=w196) -> ("error out"=w193:errorcluster)  [unwired: 8 in]
              }
              frame True {
                n56 = call "Sous_VI_recule.vi"("error in (no error)"=w199) -> ("error out"=w200:errorcluster)  [unwired: 10 in]
              }
            }
          }
          frame "Trieur" {
            # "Effectue le tri des balle en fonction de leur couleur:\nfaire tomber les balles orange"
            n57 = while {
              shift-right: [w210] -> w204
              shift-left: w202 -> [w209]
              i -> [w214]
              stop <- w212 stop-if-true
              w211 = 0.0 ("moteur gauche vite")
              n58 = Less?(x=2000, y=w214) -> (x < y?=w212:bool)
              n59 = call "Sous_VI_moteurs.vi"("error in (no error)"=w209, "Moteur Droit"=w211, "Moteur Gauche"=w211) -> ("error out"=w210:errorcluster)  [unwired: 8 in]
            }
            n60 = call "Labview_trieur_balles.vi"("error in (no error)"=w204, "Numeric"=0) -> ("error out"=w203:errorcluster)  [unwired: 9 in]
          }
          frame "Bras 2" {
            # "Bras en position pour les clapets"
            n61 = while {
              shift-right: [w221] -> w216
              shift-left: w215 -> [w220]
              i -> [w222]
              stop <- w224 stop-if-true
              n62 = Greater Or Equal?(x=w222, y=100000) -> (x >= y?=w225:bool)
              n63 = case shown="False" w225 {
                tunnel: [FALSE TRUE] -> w224
                tunnel: [w227 w230] -> w221
                tunnel: w220 -> [w226 w230]
                frame False {
                  n64 = call "Sous_VI_Bras.vi"("error in (no error)"=w226, "Enum bras"=enum_bras."Clapet Bras") -> ("error out"=w227:errorcluster)  [unwired: 9 in]
                }
                frame True {
                }
              }
            }
          }
          frame "Intersection" {
            # "Ignorer la ligne de droite"
            n65 = call "Sous_VI_acq_ligne.vi"("Seuil"=150, "error in (no error)"=w232) -> ("Décalage"=w243:u32, "G/D ?"=w234:bool, "error out"=w235:errorcluster)  [unwired: 8 in, 3 out]
            n66 = call "Sous_VI_correction.vi"("error in (no error)"=w235, "G/D ?"=w234, "Décalage"=w243) -> ("error out"=w233:errorcluster)  [unwired: 8 in]
            n67 = Select(t=Commande_1."Clapet 2", s=w237, f=Commande_1."Intersection") -> (s? t:f=w239:T2)
          }
          frame "Clapet 2" {
            # "Avance en faisant tomber les clapets avec le bras"
            n68 = call "Sous_VI_acq_ligne.vi"("Seuil"=150, "error in (no error)"=w244) -> ("Décalage"=w254:u32, "G/D ?"=w246:bool, "error out"=w247:errorcluster)  [unwired: 8 in, 3 out]
            n69 = call "Sous_VI_correction.vi"("error in (no error)"=w247, "G/D ?"=w246, "Décalage"=w254) -> ("error out"=w245:errorcluster)  [unwired: 8 in]
            n70 = Select(t=Commande_1."Monter_bras2", s=w248, f=Commande_1."Clapet 2") -> (s? t:f=w250:T2)
          }
          frame "Monter_bras2" {
            # "Monter le bras en position inactive"
            n71 = call "Sous_VI_Monter_Bras.vi"("error in (no error)"=w256) -> ("error out"=w257:errorcluster)  [unwired: 10 in]
          }
          frame "Avance3" {
            # "Avance jusqu'au virage 3"
            n72 = call "Sous_VI_acq_ligne.vi"("Seuil"=150, "error in (no error)"=w261) -> ("Décalage"=w270:u32, "G/D ?"=w264:bool, "error out"=w263:errorcluster)  [unwired: 8 in, 3 out]
            n73 = call "Sous_VI_correction.vi"("error in (no error)"=w263, "G/D ?"=w264, "Décalage"=w270) -> ("error out"=w262:errorcluster)  [unwired: 8 in]
            n74 = Select(t=Commande_1."Virage 3", s=w266, f=Commande_1."Avance3") -> (s? t:f=w267:T2)
          }
          frame "Virage 3" {
            # "Effectuer le 3 eme virage"
            n75 = call "Sous_VI_Virage_1.vi"("error in (no error)"=w273) -> ("error out"=w274:errorcluster)  [unwired: 10 in]
          }
          frame "Avance" {
            # "Avance jusqu'a la prochaine ligne à droite"
            n76 = call "Sous_VI_acq_ligne.vi"("Seuil"=150, "error in (no error)"=w278) -> ("Décalage"=w284:u32, "G/D ?"=w280:bool, "error out"=w281:errorcluster)  [unwired: 8 in, 3 out]
            n77 = call "Sous_VI_correction.vi"("error in (no error)"=w281, "G/D ?"=w280, "Décalage"=w284) -> ("error out"=w279:errorcluster)  [unwired: 8 in]
            n78 = Select(t=Commande_1."Virage 4", s=w285, f=Commande_1."Avance") -> (s? t:f=w286:T2)
          }
          frame "Virage 4" {
            # "Effectuer le 4 eme virage"
            n79 = call "Sous_VI_Virage_1.vi"("error in (no error)"=w290) -> ("error out"=w291:errorcluster)  [unwired: 10 in]
          }
          frame "Lanceur" {
            # "Se place en position devant la cible, met en route le moteur\nde la roue qui lance les balles puis le moteur du distributeur\npour lancer les balles sur la cible \nEteint les moteur"
            n80 = call "Sous_VI_Lanceur.vi"("error in (no error)"=w296, "Nb balles"=1) -> ("error out"=w295:errorcluster)  [unwired: 9 in]
          }
          frame "Demi_tour" {
            # "Faire demi tour"
            n81 = call "Sous_VI_Virage_1.vi"("error in (no error)"=w301) -> ("error out"=w302:errorcluster)  [unwired: 10 in]
          }
          frame "Virage 5" {
            # "Effectuer le 5 eme virage"
            n82 = case shown="True" w310 {
              tunnel: [Commande_1."Virage 5" Commande_1."Virage 6"] -> w311
              tunnel: [w315 w320] -> w307
              tunnel: w306 -> [w312 w319]
              frame False {
                n83 = call "Sous_VI_acq_ligne.vi"("Seuil"=150, "error in (no error)"=w312) -> ("Décalage"=w318:u32, "G/D ?"=w313:bool, "error out"=w314:errorcluster)  [unwired: 8 in, 3 out]
                n84 = call "Sous_VI_correction.vi"("error in (no error)"=w314, "G/D ?"=w313, "Décalage"=w318) -> ("error out"=w315:errorcluster)  [unwired: 8 in]
              }
              frame True {
                n85 = call "Sous_VI_Virage_cible.vi"("error in (no error)"=w319) -> ("error out"=w320:errorcluster)  [unwired: 10 in]
              }
            }
          }
          frame "Virage 6" {
            # "Effectuer le 6 eme virage"
            n86 = case shown="True" w327 {
              tunnel: [Commande_1."Virage 6" Commande_1."End"] -> w326
              tunnel: [w331 w336] -> w323
              tunnel: w322 -> [w328 w335]
              frame False {
                n87 = call "Sous_VI_acq_ligne.vi"("Seuil"=150, "error in (no error)"=w328) -> ("Décalage"=w334:u32, "G/D ?"=w329:bool, "error out"=w330:errorcluster)  [unwired: 8 in, 3 out]
                n88 = call "Sous_VI_correction.vi"("error in (no error)"=w330, "G/D ?"=w329, "Décalage"=w334) -> ("error out"=w331:errorcluster)  [unwired: 8 in]
              }
              frame True {
                n89 = call "Sous_VI_Virage_1.vi"("error in (no error)"=w335) -> ("error out"=w336:errorcluster)  [unwired: 10 in]
              }
            }
          }
          frame "End" {
            # "Changement de tour"
          }
        }
      }
      frame "Tour2" {
        n90 = case shown="\"Virage 6\"" w349 {
          tunnel: [w357 Commande_1."Clapet 1" w399 Commande_1."Avance1" w412 Commande_1."Sceaux 0" w429 w460 w486 w505 w516 w533 Commande_1."Intersection" w566 Commande_1."Clapet 2" w611 Commande_1."Avance3" w628 Commande_1."Avance" w647 Commande_1."Lanceur" Commande_1."Demi_tour" Commande_1."Virage 5" w672 w687 Commande_1."Intersection2"] -> w348
          tunnel: w344 -> [_ _ _ _ w413 _ _ _ _ w506 w515 _ _ _ _ _ _ w627 _ w646 _ _ _ w671 w688 _]
          tunnel: [T1 {"Bras"=TRUE, "Avance"=TRUE, "Tourne"=FALSE, "Sceaux"=FALSE, "Virage 2"=FALSE, "Trieur"=FALSE, "Bras 2"=FALSE, "Clapet 2"=FALSE, "Virage 3"=FALSE, "Virage 4"=FALSE, "Lanceur"=FALSE} ("Cluster 2") T1 {"Bras"=TRUE, "Avance"=TRUE, "Tourne"=FALSE, "Sceaux"=FALSE, "Virage 2"=FALSE, "Trieur"=FALSE, "Bras 2"=FALSE, "Clapet 2"=FALSE, "Virage 3"=FALSE, "Virage 4"=FALSE, "Lanceur"=FALSE} ("Cluster 2") T1 {"Bras"=TRUE, "Avance"=TRUE, "Tourne"=TRUE, "Sceaux"=FALSE, "Virage 2"=FALSE, "Trieur"=FALSE, "Bras 2"=FALSE, "Clapet 2"=FALSE, "Virage 3"=FALSE, "Virage 4"=FALSE, "Lanceur"=FALSE} ("Cluster 2") T1 {"Bras"=TRUE, "Avance"=TRUE, "Tourne"=TRUE, "Sceaux"=FALSE, "Virage 2"=FALSE, "Trieur"=FALSE, "Bras 2"=FALSE, "Clapet 2"=FALSE, "Virage 3"=FALSE, "Virage 4"=FALSE, "Lanceur"=FALSE} ("Cluster 2") T1 {"Bras"=TRUE, "Avance"=TRUE, "Tourne"=TRUE, "Sceaux"=FALSE, "Virage 2"=FALSE, "Trieur"=FALSE, "Bras 2"=FALSE, "Clapet 2"=FALSE, "Virage 3"=FALSE, "Virage 4"=FALSE, "Lanceur"=FALSE} ("Cluster 2") T1 {"Bras"=TRUE, "Avance"=TRUE, "Tourne"=TRUE, "Sceaux"=TRUE, "Virage 2"=FALSE, "Trieur"=FALSE, "Bras 2"=FALSE, "Clapet 2"=FALSE, "Virage 3"=FALSE, "Virage 4"=FALSE, "Lanceur"=FALSE} ("Cluster 2") T1 {"Bras"=TRUE, "Avance"=TRUE, "Tourne"=TRUE, "Sceaux"=TRUE, "Virage 2"=TRUE, "Trieur"=TRUE, "Bras 2"=TRUE, "Clapet 2"=TRUE, "Virage 3"=TRUE, "Virage 4"=TRUE, "Lanceur"=TRUE} ("Cluster 2") w459 w485 T1 {"Bras"=TRUE, "Avance"=TRUE, "Tourne"=TRUE, "Sceaux"=TRUE, "Virage 2"=TRUE, "Trieur"=TRUE, "Bras 2"=TRUE, "Clapet 2"=TRUE, "Virage 3"=TRUE, "Virage 4"=TRUE, "Lanceur"=TRUE} ("Cluster 2") w519 T1 {"Bras"=TRUE, "Avance"=TRUE, "Tourne"=TRUE, "Sceaux"=TRUE, "Virage 2"=TRUE, "Trieur"=FALSE, "Bras 2"=FALSE, "Clapet 2"=FALSE, "Virage 3"=FALSE, "Virage 4"=FALSE, "Lanceur"=FALSE} ("Cluster 2") T1 {"Bras"=FALSE, "Avance"=FALSE, "Tourne"=FALSE, "Sceaux"=FALSE, "Virage 2"=FALSE, "Trieur"=FALSE, "Bras 2"=FALSE, "Clapet 2"=FALSE, "Virage 3"=FALSE, "Virage 4"=FALSE, "Lanceur"=FALSE} ("Cluster 2") T1 {"Bras"=FALSE, "Avance"=FALSE, "Tourne"=FALSE, "Sceaux"=FALSE, "Virage 2"=FALSE, "Trieur"=TRUE, "Bras 2"=TRUE, "Clapet 2"=FALSE, "Virage 3"=FALSE, "Virage 4"=FALSE, "Lanceur"=FALSE} ("Cluster 2") T1 {"Bras"=FALSE, "Avance"=FALSE, "Tourne"=FALSE, "Sceaux"=FALSE, "Virage 2"=FALSE, "Trieur"=TRUE, "Bras 2"=FALSE, "Clapet 2"=FALSE, "Virage 3"=FALSE, "Virage 4"=FALSE, "Lanceur"=FALSE} ("Cluster 2") T1 {"Bras"=FALSE, "Avance"=FALSE, "Tourne"=FALSE, "Sceaux"=FALSE, "Virage 2"=FALSE, "Trieur"=TRUE, "Bras 2"=TRUE, "Clapet 2"=FALSE, "Virage 3"=FALSE, "Virage 4"=FALSE, "Lanceur"=FALSE} ("Cluster 2") T1 {"Bras"=TRUE, "Avance"=TRUE, "Tourne"=TRUE, "Sceaux"=FALSE, "Virage 2"=FALSE, "Trieur"=FALSE, "Bras 2"=FALSE, "Clapet 2"=FALSE, "Virage 3"=FALSE, "Virage 4"=FALSE, "Lanceur"=FALSE} ("Cluster 2") T1 {"Bras"=TRUE, "Avance"=TRUE, "Tourne"=TRUE, "Sceaux"=TRUE, "Virage 2"=TRUE, "Trieur"=TRUE, "Bras 2"=TRUE, "Clapet 2"=TRUE, "Virage 3"=TRUE, "Virage 4"=TRUE, "Lanceur"=TRUE} ("Cluster 2") T1 {"Bras"=FALSE, "Avance"=FALSE, "Tourne"=FALSE, "Sceaux"=FALSE, "Virage 2"=FALSE, "Trieur"=TRUE, "Bras 2"=TRUE, "Clapet 2"=TRUE, "Virage 3"=TRUE, "Virage 4"=FALSE, "Lanceur"=FALSE} ("Cluster 2") T1 {"Bras"=FALSE, "Avance"=FALSE, "Tourne"=FALSE, "Sceaux"=FALSE, "Virage 2"=FALSE, "Trieur"=FALSE, "Bras 2"=TRUE, "Clapet 2"=TRUE, "Virage 3"=TRUE, "Virage 4"=TRUE, "Lanceur"=FALSE} ("Cluster 2") T1 {"Bras"=FALSE, "Avance"=FALSE, "Tourne"=FALSE, "Sceaux"=FALSE, "Virage 2"=FALSE, "Trieur"=TRUE, "Bras 2"=TRUE, "Clapet 2"=TRUE, "Virage 3"=TRUE, "Virage 4"=TRUE, "Lanceur"=FALSE} ("Cluster 2") T1 {"Bras"=FALSE, "Avance"=FALSE, "Tourne"=FALSE, "Sceaux"=FALSE, "Virage 2"=FALSE, "Trieur"=FALSE, "Bras 2"=TRUE, "Clapet 2"=TRUE, "Virage 3"=TRUE, "Virage 4"=TRUE, "Lanceur"=TRUE} ("Cluster 2") T1 {"Bras"=FALSE, "Avance"=FALSE, "Tourne"=FALSE, "Sceaux"=FALSE, "Virage 2"=FALSE, "Trieur"=TRUE, "Bras 2"=TRUE, "Clapet 2"=TRUE, "Virage 3"=TRUE, "Virage 4"=TRUE, "Lanceur"=FALSE} ("Cluster 2") T1 {"Bras"=FALSE, "Avance"=FALSE, "Tourne"=FALSE, "Sceaux"=FALSE, "Virage 2"=FALSE, "Trieur"=TRUE, "Bras 2"=TRUE, "Clapet 2"=TRUE, "Virage 3"=TRUE, "Virage 4"=TRUE, "Lanceur"=FALSE} ("Cluster 2") T1 {"Bras"=FALSE, "Avance"=FALSE, "Tourne"=FALSE, "Sceaux"=FALSE, "Virage 2"=FALSE, "Trieur"=TRUE, "Bras 2"=TRUE, "Clapet 2"=TRUE, "Virage 3"=TRUE, "Virage 4"=TRUE, "Lanceur"=FALSE} ("Cluster 2") T1 {"Bras"=FALSE, "Avance"=FALSE, "Tourne"=FALSE, "Sceaux"=FALSE, "Virage 2"=FALSE, "Trieur"=FALSE, "Bras 2"=FALSE, "Clapet 2"=FALSE, "Virage 3"=FALSE, "Virage 4"=FALSE, "Lanceur"=FALSE} ("Cluster 2")] -> w347
          tunnel: w345 -> [w356 _ w395 _ _ _ w428 w458 w487 _ _ w534 _ w563 _ w609 _ _ _ _ _ _ _ _ _ _]
          tunnel: [enum_tour."Tour2" enum_tour."Tour2" enum_tour."Tour2" enum_tour."Tour2" enum_tour."Tour2" enum_tour."Tour2" enum_tour."Tour2" enum_tour."Tour2" enum_tour."Tour2" enum_tour."Tour2" enum_tour."Tour2" enum_tour."Tour2" enum_tour."Tour2" enum_tour."Tour2" enum_tour."Tour2" enum_tour."Tour2" enum_tour."Tour2" enum_tour."Tour2" enum_tour."Tour2" enum_tour."Tour2" enum_tour."Tour2" enum_tour."Tour2" enum_tour."Tour2" enum_tour."Tour2" enum_tour."Tour2" enum_tour."Tour3"] -> w346
          tunnel: w343 -> [w351 w365 w390 w402 w407 w419 w424 w455 w483 w500 w512 w530 w546 w560 w574 w605 w617 w622 w634 w639 w651 w656 w662 w667 w683 w698]
          tunnel: [w350 w362 w391 w403 w408 w420 w425 w456 w482 w501 w513 w531 w548 w559 w571 w606 w618 w623 w635 w640 w652 w657 w663 w668 w684 w698] -> w342
          frame "Intersection2", Default {
            # "Ignore la 1 ere intersection a gauche"
            n91 = call "Sous_VI_acq_ligne.vi"("Seuil"=150, "error in (no error)"=w351) -> ("Décalage"=w355:u32, "G/D ?"=w353:bool, "error out"=w352:errorcluster)  [unwired: 8 in, 3 out]
            n92 = call "Sous_VI_correction.vi"("error in (no error)"=w352, "G/D ?"=w353, "Décalage"=w355) -> ("error out"=w350:errorcluster)  [unwired: 8 in]
            n93 = Select(t=Commande_1."Bras", s=w356, f=Commande_1."Intersection2") -> (s? t:f=w357:T2)
          }
          frame "Bras" {
            # "Baisser le bras pour faire tomber le 2 eme clapet"
            n94 = while {
              shift-right: [w381] -> w364
              shift-left: w365 -> [w382]
              i -> [w389]
              stop <- w387 stop-if-true
              n95 = Less?(x=1500, y=w389) -> (x < y?=w387:bool)
              n96 = call "Sous_VI_acq_ligne.vi"("Seuil"=150, "error in (no error)"=w382) -> ("Décalage"=w385:u32, "G/D ?"=w384:bool, "error out"=w383:errorcluster)  [unwired: 8 in, 3 out]
              n97 = call "Sous_VI_correction.vi"("error in (no error)"=w383, "G/D ?"=w384, "Décalage"=w385) -> ("error out"=w381:errorcluster)  [unwired: 8 in]
            }
            n98 = while {
              shift-right: [w375] -> w363
              shift-left: w364 -> [w376]
              i -> [w380]
              stop <- w378 stop-if-true
              w377 = 0.0 ("moteur gauche vite")
              n99 = call "Sous_VI_moteurs.vi"("error in (no error)"=w376, "Moteur Droit"=w377, "Moteur Gauche"=w377) -> ("error out"=w375:errorcluster)  [unwired: 8 in]
              n100 = Less?(x=1500, y=w380) -> (x < y?=w378:bool)
            }
            n101 = while {
              shift-right: [w369] -> w362
              shift-left: w363 -> [w370]
              i -> [w374]
              stop <- w372 stop-if-true
              n102 = Less?(x=1500, y=w374) -> (x < y?=w372:bool)
              n103 = call "Sous_VI_Bras.vi"("error in (no error)"=w370, "Enum bras"=enum_bras."Clapet Bras") -> ("error out"=w369:errorcluster)  [unwired: 9 in]
            }
          }
          frame "Clapet 1" {
            # "Faire tomber le 2 eme clapet"
            n104 = call "Sous_VI_acq_ligne.vi"("Seuil"=150, "error in (no error)"=w390) -> ("Décalage"=w397:u32, "G/D ?"=w393:bool, "error out"=w392:errorcluster)  [unwired: 8 in, 3 out]
            n105 = call "Sous_VI_correction.vi"("error in (no error)"=w392, "G/D ?"=w393, "Décalage"=w397) -> ("error out"=w391:errorcluster)  [unwired: 8 in]
            n106 = Select(t=Commande_1."Monter_bras1", s=w395, f=Commande_1."Clapet 1") -> (s? t:f=w399:T2)
          }
          frame "Monter_bras1" {
            # "Monter le bras après le clapet 2"
            n107 = call "Sous_VI_Monter_Bras.vi"("error in (no error)"=w402) -> ("error out"=w403:errorcluster)  [unwired: 10 in]
          }
          frame "Avance1" {
            # "Avancer jusqu'au virage 1"
            n108 = call "Sous_VI_acq_ligne.vi"("Seuil"=150, "error in (no error)"=w407) -> ("Décalage"=w415:u32, "G/D ?"=w409:bool, "error out"=w410:errorcluster)  [unwired: 8 in, 3 out]
            n109 = call "Sous_VI_correction.vi"("error in (no error)"=w410, "G/D ?"=w409, "Décalage"=w415) -> ("error out"=w408:errorcluster)  [unwired: 8 in]
            n110 = Select(t=Commande_1."Virage 1", s=w413, f=Commande_1."Avance1") -> (s? t:f=w412:T2)
          }
          frame "Virage 1" {
            # "Effectuer le 1 er virage"
            n111 = call "Sous_VI_Virage_1.vi"("error in (no error)"=w419) -> ("error out"=w420:errorcluster)  [unwired: 10 in]
          }
          frame "Sceaux 0" {
            # "Se placer de sorte d'ignorer la première ligne à gauche"
            n112 = case shown="True" w428 {
              tunnel: [Commande_1."Sceaux 0" Commande_1."Sceaux 1"] -> w429
              tunnel: [w431 w437] -> w425
              tunnel: w424 -> [w430 w438]
              frame False {
                n113 = call "Sous_VI_acq_ligne.vi"("Seuil"=150, "error in (no error)"=w430) -> ("Décalage"=w435:u32, "G/D ?"=w433:bool, "error out"=w432:errorcluster)  [unwired: 8 in, 3 out]
                n114 = call "Sous_VI_correction.vi"("error in (no error)"=w432, "G/D ?"=w433, "Décalage"=w435) -> ("error out"=w431:errorcluster)  [unwired: 8 in]
              }
              frame True {
                n115 = while {
                  shift-right: [w440] -> w437
                  shift-left: w438 -> [w441]
                  i -> [w445]
                  stop <- w442 stop-if-true
                  n116 = Greater Or Equal?(x=w445, y=200) -> (x >= y?=w443:bool)
                  n117 = case shown="False" w443 {
                    tunnel: [FALSE TRUE] -> w442
                    tunnel: w441 -> [w447 w453]
                    tunnel: [w446 w453] -> w440
                    frame False {
                      n118 = call "Sous_VI_acq_ligne.vi"("Seuil"=150, "error in (no error)"=w447) -> ("Décalage"=w452:u32, "G/D ?"=w449:bool, "error out"=w448:errorcluster)  [unwired: 8 in, 3 out]
                      n119 = call "Sous_VI_correction.vi"("error in (no error)"=w448, "G/D ?"=w449, "Décalage"=w452) -> ("error out"=w446:errorcluster)  [unwired: 8 in]
                    }
                    frame True {
                    }
                  }
                }
              }
            }
          }
          frame "Sceaux 1" {
            # "Ignore le sceaux 1"
            n120 = case shown="True" w458 {
              tunnel: [T1 {"Bras"=TRUE, "Avance"=TRUE, "Tourne"=TRUE, "Sceaux"=FALSE, "Virage 2"=FALSE, "Trieur"=FALSE, "Bras 2"=FALSE, "Clapet 2"=FALSE, "Virage 3"=FALSE, "Virage 4"=FALSE, "Lanceur"=FALSE} ("Cluster 2") T1 {"Bras"=TRUE, "Avance"=TRUE, "Tourne"=TRUE, "Sceaux"=TRUE, "Virage 2"=TRUE, "Trieur"=TRUE, "Bras 2"=TRUE, "Clapet 2"=TRUE, "Virage 3"=TRUE, "Virage 4"=TRUE, "Lanceur"=TRUE} ("Cluster 2")] -> w459
              tunnel: [w464 w471] -> w456
              tunnel: w455 -> [w463 w470]
              frame False {
                n121 = call "Sous_VI_acq_ligne.vi"("Seuil"=150, "error in (no error)"=w463) -> ("Décalage"=w468:u32, "G/D ?"=w466:bool, "error out"=w465:errorcluster)  [unwired: 8 in, 3 out]
                n122 = call "Sous_VI_correction.vi"("error in (no error)"=w465, "G/D ?"=w466, "Décalage"=w468) -> ("error out"=w464:errorcluster)  [unwired: 8 in]
              }
              frame True {
                n123 = while {
                  shift-right: [w474] -> w471
                  shift-left: w470 -> [w473]
                  i -> [w481]
                  stop <- w477 stop-if-true
                  n124 = call "Sous_VI_acq_ligne.vi"("Seuil"=150, "error in (no error)"=w473) -> ("Décalage"=w478:u32, "G/D ?"=w475:bool, "error out"=w476:errorcluster)  [unwired: 8 in, 3 out]
                  n125 = Greater Or Equal?(x=w481, y=200) -> (x >= y?=w477:bool)
                  n126 = call "Sous_VI_correction.vi"("error in (no error)"=w476, "G/D ?"=w475, "Décalage"=w478) -> ("error out"=w474:errorcluster)  [unwired: 8 in]
                }
              }
            }
            n127 = Select(t=Commande_1."Sceaux 2", s=w458, f=Commande_1."Sceaux 1") -> (s? t:f=w460:T2)
          }
          frame "Sceaux 2" {
            # "Tapper la balle sur le sceau 2 avec le bras"
            n128 = case shown="True" w487 {
              tunnel: [T1 {"Bras"=TRUE, "Avance"=TRUE, "Tourne"=TRUE, "Sceaux"=FALSE, "Virage 2"=FALSE, "Trieur"=FALSE, "Bras 2"=FALSE, "Clapet 2"=FALSE, "Virage 3"=FALSE, "Virage 4"=FALSE, "Lanceur"=FALSE} ("Cluster 2") T1 {"Bras"=TRUE, "Avance"=TRUE, "Tourne"=TRUE, "Sceaux"=TRUE, "Virage 2"=TRUE, "Trieur"=TRUE, "Bras 2"=TRUE, "Clapet 2"=TRUE, "Virage 3"=TRUE, "Virage 4"=TRUE, "Lanceur"=TRUE} ("Cluster 2")] -> w485
              tunnel: w483 -> [w490 w498]
              tunnel: [w491 w497] -> w482
              frame False {
                n129 = call "Sous_VI_acq_ligne.vi"("Seuil"=150, "error in (no error)"=w490) -> ("Décalage"=w495:u32, "G/D ?"=w492:bool, "error out"=w493:errorcluster)  [unwired: 8 in, 3 out]
                n130 = call "Sous_VI_correction.vi"("error in (no error)"=w493, "G/D ?"=w492, "Décalage"=w495) -> ("error out"=w491:errorcluster)  [unwired: 8 in]
              }
              frame True {
                n131 = call "Sous_VI_Sceaux.vi"("error in (no error)"=w498) -> ("error out"=w497:errorcluster)  [unwired: 10 in]
              }
            }
            n132 = Select(t=Commande_1."Virage 2", s=w487, f=Commande_1."Sceaux 2") -> (s? t:f=w486:T2)
          }
          frame "Avance2" {
            # "Avance jusqu'au virage 2"
            n133 = call "Sous_VI_acq_ligne.vi"("Seuil"=150, "error in (no error)"=w500) -> ("Décalage"=w508:u32, "G/D ?"=w503:bool, "error out"=w502:errorcluster)  [unwired: 8 in, 3 out]
            n134 = call "Sous_VI_correction.vi"("error in (no error)"=w502, "G/D ?"=w503, "Décalage"=w508) -> ("error out"=w501:errorcluster)  [unwired: 8 in]
            n135 = Select(t=Commande_1."Virage 2", s=w506, f=Commande_1."Avance2") -> (s? t:f=w505:T2)
          }
          frame "Virage 2" {
            # "Effectuer le 2 eme virage"
            n136 = case shown="True" w515 {
              tunnel: [T1 {"Bras"=TRUE, "Avance"=TRUE, "Tourne"=TRUE, "Sceaux"=FALSE, "Virage 2"=FALSE, "Trieur"=FALSE, "Bras 2"=FALSE, "Clapet 2"=FALSE, "Virage 3"=FALSE, "Virage 4"=FALSE, "Lanceur"=FALSE} ("Cluster 2") T1 {"Bras"=TRUE, "Avance"=TRUE, "Tourne"=TRUE, "Sceaux"=TRUE, "Virage 2"=FALSE, "Trieur"=FALSE, "Bras 2"=FALSE, "Clapet 2"=FALSE, "Virage 3"=FALSE, "Virage 4"=FALSE, "Lanceur"=FALSE} ("Cluster 2")] -> w519
              tunnel: [w521 w528] -> w513
              tunnel: w512 -> [w520 w527]
              frame False {
                n137 = call "Sous_VI_acq_ligne.vi"("Seuil"=150, "error in (no error)"=w520) -> ("Décalage"=w525:u32, "G/D ?"=w522:bool, "error out"=w523:errorcluster)  [unwired: 8 in, 3 out]
                n138 = call "Sous_VI_correction.vi"("error in (no error)"=w523, "G/D ?"=w522, "Décalage"=w525) -> ("error out"=w521:errorcluster)  [unwired: 8 in]
              }
              frame True {
                n139 = call "Sous_VI_Virage_1.vi"("error in (no error)"=w527) -> ("error out"=w528:errorcluster)  [unwired: 10 in]
              }
            }
            n140 = Select(t=Commande_1."Recule", s=w515, f=Commande_1."Virage 2") -> (s? t:f=w516:T2)
          }
          frame "Recule" {
            # "Avance jusqu'à la ligne de gauche \npuis recule jusqu'à la zone de tri"
            n141 = case shown="True" w534 {
              tunnel: [Commande_1."Recule" Commande_1."Trieur"] -> w533
              tunnel: [w537 w544] -> w531
              tunnel: w530 -> [w536 w543]
              frame False {
                n142 = call "Sous_VI_acq_ligne.vi"("Seuil"=150, "error in (no error)"=w536) -> ("Décalage"=w540:u32, "G/D ?"=w539:bool, "error out"=w538:errorcluster)  [unwired: 8 in, 3 out]
                n143 = call "Sous_VI_correction.vi"("error in (no error)"=w538, "G/D ?"=w539, "Décalage"=w540) -> ("error out"=w537:errorcluster)  [unwired: 8 in]
              }
              frame True {
                n144 = call "Sous_VI_recule.vi"("error in (no error)"=w543) -> ("error out"=w544:errorcluster)  [unwired: 10 in]
              }
            }
          }
          frame "Trieur" {
            # "Effectue le tri des balle en fonction de leur couleur:\nfaire tomber les balles orange"
            n145 = while {
              shift-right: [w554] -> w547
              shift-left: w546 -> [w553]
              i -> [w558]
              stop <- w556 stop-if-true
              w555 = 0.0 ("moteur gauche vite")
              n146 = Less?(x=2000, y=w558) -> (x < y?=w556:bool)
              n147 = call "Sous_VI_moteurs.vi"("error in (no error)"=w553, "Moteur Droit"=w555, "Moteur Gauche"=w555) -> ("error out"=w554:errorcluster)  [unwired: 8 in]
            }
            n148 = call "Labview_trieur_balles.vi"("error in (no error)"=w547, "Numeric"=2) -> ("error out"=w548:errorcluster)  [unwired: 9 in]
          }
          frame "Intersection" {
            # "Ignore la 1 ere ligne a gauche"
            n149 = call "Sous_VI_acq_ligne.vi"("Seuil"=150, "error in (no error)"=w560) -> ("Décalage"=w570:u32, "G/D ?"=w562:bool, "error out"=w561:errorcluster)  [unwired: 8 in, 3 out]
            n150 = call "Sous_VI_correction.vi"("error in (no error)"=w561, "G/D ?"=w562, "Décalage"=w570) -> ("error out"=w559:errorcluster)  [unwired: 8 in]
            n151 = Select(t=Commande_1."Bras 2", s=w563, f=Commande_1."Intersection") -> (s? t:f=w566:T2)
          }
          frame "Bras 2" {
            # "Bras en position pour les clapets"
            n152 = while {
              shift-right: [w596] -> w573
              shift-left: w574 -> [w597]
              i -> [w604]
              stop <- w602 stop-if-true
              n153 = call "Sous_VI_acq_ligne.vi"("Seuil"=150, "error in (no error)"=w597) -> ("Décalage"=w601:u32, "G/D ?"=w599:bool, "error out"=w598:errorcluster)  [unwired: 8 in, 3 out]
              n154 = Less?(x=1500, y=w604) -> (x < y?=w602:bool)
              n155 = call "Sous_VI_correction.vi"("error in (no error)"=w598, "G/D ?"=w599, "Décalage"=w601) -> ("error out"=w596:errorcluster)  [unwired: 8 in]
            }
            n156 = while {
              shift-right: [w590] -> w572
              shift-left: w573 -> [w591]
              i -> [w595]
              stop <- w593 stop-if-true
              w592 = 0.0 ("moteur gauche vite")
              n157 = call "Sous_VI_moteurs.vi"("error in (no error)"=w591, "Moteur Droit"=w592, "Moteur Gauche"=w592) -> ("error out"=w590:errorcluster)  [unwired: 8 in]
              n158 = Less?(x=1500, y=w595) -> (x < y?=w593:bool)
            }
            n159 = while {
              shift-right: [w578] -> w571
              shift-left: w572 -> [w579]
              i -> [w580]
              stop <- w582 stop-if-true
              n160 = Greater Or Equal?(x=w580, y=1500) -> (x >= y?=w583:bool)
              n161 = case shown="False" w583 {
                tunnel: [FALSE TRUE] -> w582
                tunnel: w579 -> [w585 w588]
                tunnel: [w584 w588] -> w578
                frame False {
                  n162 = call "Sous_VI_Bras.vi"("error in (no error)"=w585, "Enum bras"=enum_bras."Clapet Bras") -> ("error out"=w584:errorcluster)  [unwired: 9 in]
                }
                frame True {
                }
              }
            }
          }
          frame "Clapet 2" {
            # "Avance en faisant tomber les clapets avec le bras"
            n163 = call "Sous_VI_acq_ligne.vi"("Seuil"=150, "error in (no error)"=w605) -> ("Décalage"=w615:u32, "G/D ?"=w608:bool, "error out"=w607:errorcluster)  [unwired: 8 in, 3 out]
            n164 = call "Sous_VI_correction.vi"("error in (no error)"=w607, "G/D ?"=w608, "Décalage"=w615) -> ("error out"=w606:errorcluster)  [unwired: 8 in]
            n165 = Select(t=Commande_1."Monter_bras2", s=w609, f=Commande_1."Clapet 2") -> (s? t:f=w611:T2)
          }
          frame "Monter_bras2" {
            # "Monter le bras en position inactive"
            n166 = call "Sous_VI_Monter_Bras.vi"("error in (no error)"=w617) -> ("error out"=w618:errorcluster)  [unwired: 10 in]
          }
          frame "Avance3" {
            # "Avance jusqu'au virage 3"
            n167 = call "Sous_VI_acq_ligne.vi"("Seuil"=150, "error in (no error)"=w622) -> ("Décalage"=w631:u32, "G/D ?"=w625:bool, "error out"=w624:errorcluster)  [unwired: 8 in, 3 out]
            n168 = call "Sous_VI_correction.vi"("error in (no error)"=w624, "G/D ?"=w625, "Décalage"=w631) -> ("error out"=w623:errorcluster)  [unwired: 8 in]
            n169 = Select(t=Commande_1."Virage 3", s=w627, f=Commande_1."Avance3") -> (s? t:f=w628:T2)
          }
          frame "Virage 3" {
            # "Effectuer le 3 eme virage"
            n170 = call "Sous_VI_Virage_1.vi"("error in (no error)"=w634) -> ("error out"=w635:errorcluster)  [unwired: 10 in]
          }
          frame "Avance" {
            # "Avance jusqu'a la prochaine ligne à droite"
            n171 = call "Sous_VI_acq_ligne.vi"("Seuil"=150, "error in (no error)"=w639) -> ("Décalage"=w645:u32, "G/D ?"=w642:bool, "error out"=w641:errorcluster)  [unwired: 8 in, 3 out]
            n172 = call "Sous_VI_correction.vi"("error in (no error)"=w641, "G/D ?"=w642, "Décalage"=w645) -> ("error out"=w640:errorcluster)  [unwired: 8 in]
            n173 = Select(t=Commande_1."Virage 4", s=w646, f=Commande_1."Avance") -> (s? t:f=w647:T2)
          }
          frame "Virage 4" {
            # "Effectuer le 4 eme virage"
            n174 = call "Sous_VI_Virage_1.vi"("error in (no error)"=w651) -> ("error out"=w652:errorcluster)  [unwired: 10 in]
          }
          frame "Lanceur" {
            # "Se place en position devant la cible, met en route le moteur\nde la roue qui lance les balles puis le moteur du distributeur\npour lancer les balles sur la cible \nEteint les moteur"
            n175 = call "Sous_VI_Lanceur.vi"("error in (no error)"=w656, "Nb balles"=1) -> ("error out"=w657:errorcluster)  [unwired: 9 in]
          }
          frame "Demi_tour" {
            # "Faire demi tour"
            n176 = call "Sous_VI_Virage_1.vi"("error in (no error)"=w662) -> ("error out"=w663:errorcluster)  [unwired: 10 in]
          }
          frame "Virage 5" {
            # "Effectuer le 5 eme virage"
            n177 = case shown="False" w671 {
              tunnel: [Commande_1."Virage 5" Commande_1."Virage 6"] -> w672
              tunnel: [w674 w681] -> w668
              tunnel: w667 -> [w673 w680]
              frame False {
                n178 = call "Sous_VI_acq_ligne.vi"("Seuil"=150, "error in (no error)"=w673) -> ("Décalage"=w679:u32, "G/D ?"=w676:bool, "error out"=w675:errorcluster)  [unwired: 8 in, 3 out]
                n179 = call "Sous_VI_correction.vi"("error in (no error)"=w675, "G/D ?"=w676, "Décalage"=w679) -> ("error out"=w674:errorcluster)  [unwired: 8 in]
              }
              frame True {
                n180 = call "Sous_VI_Virage_cible.vi"("error in (no error)"=w680) -> ("error out"=w681:errorcluster)  [unwired: 10 in]
              }
            }
          }
          frame "Virage 6" {
            # "Effectuer le 6 eme virage"
            n181 = case shown="True" w688 {
              tunnel: [Commande_1."Virage 6" Commande_1."End"] -> w687
              tunnel: [w689 w696] -> w684
              tunnel: w683 -> [_ w695]
              frame False {
                n182 = call "Sous_VI_acq_ligne.vi"("Seuil"=150) -> ("Décalage"=w694:u32, "G/D ?"=w691:bool, "error out"=w690:errorcluster)  [unwired: 9 in, 3 out]
                n183 = call "Sous_VI_correction.vi"("error in (no error)"=w690, "G/D ?"=w691, "Décalage"=w694) -> ("error out"=w689:errorcluster)  [unwired: 8 in]
              }
              frame True {
                n184 = call "Sous_VI_Virage_1.vi"("error in (no error)"=w695) -> ("error out"=w696:errorcluster)  [unwired: 10 in]
              }
            }
          }
          frame "End" {
            # "Changement de tour"
          }
        }
      }
      frame "Tour3" {
        n185 = case shown="\"Virage 3\"" w704 {
          tunnel: [w713 w742 Commande_1."Clapet 1" w775 Commande_1."Sceaux 0" w787 w818 w845 w869 Commande_1."Virage 2" w915 w932 Commande_1."Intersection" w963 w990 Commande_1."Clapet 2" w1019 Commande_1."Avance" w1058 Commande_1."Lanceur" Commande_1."Demi_tour" Commande_1."Virage 5" w1083 w1098 Commande_1."End"] -> w709
          tunnel: w705 -> [_ _ _ w770 _ _ _ _ _ _ w914 _ _ _ _ _ w1017 _ w1057 _ _ _ w1082 w1099 _]
          tunnel: [T1 {"Bras"=TRUE, "Avance"=TRUE, "Tourne"=FALSE, "Sceaux"=FALSE, "Virage 2"=FALSE, "Trieur"=FALSE, "Bras 2"=FALSE, "Clapet 2"=FALSE, "Virage 3"=FALSE, "Virage 4"=FALSE, "Lanceur"=FALSE} ("Cluster 2") T1 {"Bras"=TRUE, "Avance"=TRUE, "Tourne"=FALSE, "Sceaux"=FALSE, "Virage 2"=FALSE, "Trieur"=FALSE, "Bras 2"=FALSE, "Clapet 2"=FALSE, "Virage 3"=FALSE, "Virage 4"=FALSE, "Lanceur"=FALSE} ("Cluster 2") T1 {"Bras"=TRUE, "Avance"=TRUE, "Tourne"=FALSE, "Sceaux"=FALSE, "Virage 2"=FALSE, "Trieur"=FALSE, "Bras 2"=FALSE, "Clapet 2"=FALSE, "Virage 3"=FALSE, "Virage 4"=FALSE, "Lanceur"=FALSE} ("Cluster 2") T1 {"Bras"=TRUE, "Avance"=TRUE, "Tourne"=TRUE, "Sceaux"=FALSE, "Virage 2"=FALSE, "Trieur"=FALSE, "Bras 2"=FALSE, "Clapet 2"=FALSE, "Virage 3"=FALSE, "Virage 4"=FALSE, "Lanceur"=FALSE} ("Cluster 2") T1 {"Bras"=TRUE, "Avance"=TRUE, "Tourne"=TRUE, "Sceaux"=TRUE, "Virage 2"=FALSE, "Trieur"=FALSE, "Bras 2"=FALSE, "Clapet 2"=FALSE, "Virage 3"=FALSE, "Virage 4"=FALSE, "Lanceur"=FALSE} ("Cluster 2") T1 {"Bras"=TRUE, "Avance"=TRUE, "Tourne"=TRUE, "Sceaux"=TRUE, "Virage 2"=TRUE, "Trieur"=TRUE, "Bras 2"=TRUE, "Clapet 2"=TRUE, "Virage 3"=TRUE, "Virage 4"=TRUE, "Lanceur"=TRUE} ("Cluster 2") w817 w843 w871 T1 {"Bras"=TRUE, "Avance"=TRUE, "Tourne"=TRUE, "Sceaux"=TRUE, "Virage 2"=TRUE, "Trieur"=TRUE, "Bras 2"=TRUE, "Clapet 2"=TRUE, "Virage 3"=TRUE, "Virage 4"=TRUE, "Lanceur"=TRUE} ("Cluster 2") w918 T1 {"Bras"=TRUE, "Avance"=TRUE, "Tourne"=TRUE, "Sceaux"=TRUE, "Virage 2"=TRUE, "Trieur"=FALSE, "Bras 2"=FALSE, "Clapet 2"=FALSE, "Virage 3"=FALSE, "Virage 4"=FALSE, "Lanceur"=FALSE} ("Cluster 2") T1 {"Bras"=FALSE, "Avance"=FALSE, "Tourne"=FALSE, "Sceaux"=FALSE, "Virage 2"=FALSE, "Trieur"=FALSE, "Bras 2"=FALSE, "Clapet 2"=FALSE, "Virage 3"=FALSE, "Virage 4"=FALSE, "Lanceur"=FALSE} ("Cluster 2") T1 {"Bras"=FALSE, "Avance"=FALSE, "Tourne"=FALSE, "Sceaux"=FALSE, "Virage 2"=FALSE, "Trieur"=TRUE, "Bras 2"=TRUE, "Clapet 2"=FALSE, "Virage 3"=FALSE, "Virage 4"=FALSE, "Lanceur"=FALSE} ("Cluster 2") T1 {"Bras"=FALSE, "Avance"=FALSE, "Tourne"=FALSE, "Sceaux"=FALSE, "Virage 2"=FALSE, "Trieur"=TRUE, "Bras 2"=TRUE, "Clapet 2"=FALSE, "Virage 3"=FALSE, "Virage 4"=FALSE, "Lanceur"=FALSE} ("Cluster 2") T1 {"Bras"=FALSE, "Avance"=FALSE, "Tourne"=FALSE, "Sceaux"=FALSE, "Virage 2"=FALSE, "Trieur"=TRUE, "Bras 2"=FALSE, "Clapet 2"=FALSE, "Virage 3"=FALSE, "Virage 4"=FALSE, "Lanceur"=FALSE} ("Cluster 2") T1 {"Bras"=FALSE, "Avance"=FALSE, "Tourne"=FALSE, "Sceaux"=FALSE, "Virage 2"=FALSE, "Trieur"=TRUE, "Bras 2"=TRUE, "Clapet 2"=FALSE, "Virage 3"=FALSE, "Virage 4"=FALSE, "Lanceur"=FALSE} ("Cluster 2") T1 {"Bras"=FALSE, "Avance"=FALSE, "Tourne"=FALSE, "Sceaux"=FALSE, "Virage 2"=FALSE, "Trieur"=TRUE, "Bras 2"=TRUE, "Clapet 2"=TRUE, "Virage 3"=TRUE, "Virage 4"=FALSE, "Lanceur"=FALSE} ("Cluster 2") T1 {"Bras"=FALSE, "Avance"=FALSE, "Tourne"=FALSE, "Sceaux"=FALSE, "Virage 2"=FALSE, "Trieur"=FALSE, "Bras 2"=TRUE, "Clapet 2"=TRUE, "Virage 3"=TRUE, "Virage 4"=TRUE, "Lanceur"=FALSE} ("Cluster 2") T1 {"Bras"=FALSE, "Avance"=FALSE, "Tourne"=FALSE, "Sceaux"=FALSE, "Virage 2"=FALSE, "Trieur"=TRUE, "Bras 2"=TRUE, "Clapet 2"=TRUE, "Virage 3"=TRUE, "Virage 4"=TRUE, "Lanceur"=FALSE} ("Cluster 2") T1 {"Bras"=FALSE, "Avance"=FALSE, "Tourne"=FALSE, "Sceaux"=FALSE, "Virage 2"=FALSE, "Trieur"=FALSE, "Bras 2"=TRUE, "Clapet 2"=TRUE, "Virage 3"=TRUE, "Virage 4"=TRUE, "Lanceur"=TRUE} ("Cluster 2") T1 {"Bras"=FALSE, "Avance"=FALSE, "Tourne"=FALSE, "Sceaux"=FALSE, "Virage 2"=FALSE, "Trieur"=TRUE, "Bras 2"=TRUE, "Clapet 2"=TRUE, "Virage 3"=TRUE, "Virage 4"=TRUE, "Lanceur"=FALSE} ("Cluster 2") T1 {"Bras"=FALSE, "Avance"=FALSE, "Tourne"=FALSE, "Sceaux"=FALSE, "Virage 2"=FALSE, "Trieur"=TRUE, "Bras 2"=TRUE, "Clapet 2"=TRUE, "Virage 3"=TRUE, "Virage 4"=TRUE, "Lanceur"=FALSE} ("Cluster 2") T1 {"Bras"=FALSE, "Avance"=FALSE, "Tourne"=FALSE, "Sceaux"=FALSE, "Virage 2"=FALSE, "Trieur"=TRUE, "Bras 2"=TRUE, "Clapet 2"=TRUE, "Virage 3"=TRUE, "Virage 4"=TRUE, "Lanceur"=FALSE} ("Cluster 2") T1 {"Bras"=FALSE, "Avance"=FALSE, "Tourne"=FALSE, "Sceaux"=FALSE, "Virage 2"=FALSE, "Trieur"=FALSE, "Bras 2"=FALSE, "Clapet 2"=FALSE, "Virage 3"=FALSE, "Virage 4"=FALSE, "Lanceur"=FALSE} ("Cluster 2")] -> w708
          tunnel: w706 -> [w712 w743 _ _ _ w786 w816 w842 w872 _ _ w933 _ w960 w991 _ _ _ _ _ _ _ _ _ _]
          tunnel: [enum_tour."Tour3" enum_tour."Tour3" enum_tour."Tour3" enum_tour."Tour3" enum_tour."Tour3" enum_tour."Tour3" enum_tour."Tour3" enum_tour."Tour3" enum_tour."Tour3" enum_tour."Tour3" enum_tour."Tour3" enum_tour."Tour3" enum_tour."Tour3" enum_tour."Tour3" enum_tour."Tour3" enum_tour."Tour3" enum_tour."Tour3" enum_tour."Tour3" enum_tour."Tour3" enum_tour."Tour3" enum_tour."Tour3" enum_tour."Tour3" enum_tour."Tour3" enum_tour."Tour3" enum_tour."Tour3"] -> w707
          tunnel: w703 -> [w711 w736 w747 w765 w777 w783 w813 w841 w867 w885 w911 w929 w945 w959 w983 w995 w1013 w1028 w1050 w1062 w1067 w1073 w1078 w1094 w1111]
          tunnel: [w710 w735 w749 w766 w778 w782 w814 w840 w868 w886 w912 w930 w946 w958 w984 w996 w1014 w1025 w1051 w1063 w1068 w1074 w1079 w1095 w1110] -> w702
          frame "Intersection2", Default {
            # "Ignore la 1 ere intersection a gauche"
            n186 = case shown="True" w712 {
              tunnel: w711 -> [w718 w725]
              tunnel: [w719 w724] -> w710
              frame False {
                n187 = call "Sous_VI_acq_ligne.vi"("Seuil"=150, "error in (no error)"=w718) -> ("Décalage"=w722:u32, "G/D ?"=w721:bool, "error out"=w720:errorcluster)  [unwired: 8 in, 3 out]
                n188 = call "Sous_VI_correction.vi"("error in (no error)"=w720, "G/D ?"=w721, "Décalage"=w722) -> ("error out"=w719:errorcluster)  [unwired: 8 in]
              }
              frame True {
                n189 = while {
                  shift-right: [w726] -> w724
                  shift-left: w725 -> [w727]
                  i -> [w734]
                  stop <- w730 stop-if-true
                  n190 = call "Sous_VI_acq_ligne.vi"("Seuil"=150, "error in (no error)"=w727) -> ("Décalage"=w731:u32, "G/D ?"=w729:bool, "error out"=w728:errorcluster)  [unwired: 8 in, 3 out]
                  n191 = Greater Or Equal?(x=w734, y=200) -> (x >= y?=w730:bool)
                  n192 = call "Sous_VI_correction.vi"("error in (no error)"=w728, "G/D ?"=w729, "Décalage"=w731) -> ("error out"=w726:errorcluster)  [unwired: 8 in]
                }
              }
            }
            n193 = Select(t=Commande_1."Intersection3", s=w712, f=Commande_1."Intersection2") -> (s? t:f=w713:T2)
          }
          frame "Intersection3" {
            # "Ignore la 2 eme intersection a gauche"
            n194 = call "Sous_VI_acq_ligne.vi"("Seuil"=150, "error in (no error)"=w736) -> ("Décalage"=w745:u32, "G/D ?"=w738:bool, "error out"=w737:errorcluster)  [unwired: 8 in, 3 out]
            n195 = call "Sous_VI_correction.vi"("error in (no error)"=w737, "G/D ?"=w738, "Décalage"=w745) -> ("error out"=w735:errorcluster)  [unwired: 8 in]
            n196 = Select(t=Commande_1."Bras", s=w743, f=Commande_1."Intersection3") -> (s? t:f=w742:T2)
          }
          frame "Bras" {
            w751 = 0.0 ("moteur gauche vite")
            # "Baisser le bras pour faire tomber le 3 eme clapet"
            n197 = while {
              shift-right: [w757] -> w748
              shift-left: w747 -> [w756]
              i -> [w764]
              stop <- w762 stop-if-true
              n198 = Less?(x=1500, y=w764) -> (x < y?=w762:bool)
              n199 = call "Sous_VI_acq_ligne.vi"("Seuil"=150, "error in (no error)"=w756) -> ("Décalage"=w760:u32, "G/D ?"=w759:bool, "error out"=w758:errorcluster)  [unwired: 8 in, 3 out]
              n200 = call "Sous_VI_correction.vi"("error in (no error)"=w758, "G/D ?"=w759, "Décalage"=w760) -> ("error out"=w757:errorcluster)  [unwired: 8 in]
            }
            n201 = call "Sous_VI_moteurs.vi"("error in (no error)"=w748, "Moteur Droit"=w751, "Moteur Gauche"=w751) -> ("error out"=w750:errorcluster)  [unwired: 8 in]
            n202 = call "Sous_VI_Bras.vi"("error in (no error)"=w750, "Enum bras"=enum_bras."Clapet Bras") -> ("error out"=w749:errorcluster)  [unwired: 9 in]
          }
          frame "Clapet 1" {
            # "Faire tomber le 3 eme clapet"
            n203 = call "Sous_VI_acq_ligne.vi"("Seuil"=150, "error in (no error)"=w765) -> ("Décalage"=w773:u32, "G/D ?"=w768:bool, "error out"=w767:errorcluster)  [unwired: 8 in, 3 out]
            n204 = call "Sous_VI_correction.vi"("error in (no error)"=w767, "G/D ?"=w768, "Décalage"=w773) -> ("error out"=w766:errorcluster)  [unwired: 8 in]
            n205 = Select(t=Commande_1."Virage 1", s=w770, f=Commande_1."Clapet 1") -> (s? t:f=w775:T2)
          }
          frame "Virage 1" {
            # "Effectuer le 1 er virage"
            n206 = call "Sous_VI_Virage_1.vi"("error in (no error)"=w777) -> ("error out"=w778:errorcluster)  [unwired: 10 in]
          }
          frame "Sceaux 0" {
            # "Se placer de sorte d'ignorer la première ligne à gauche"
            n207 = case shown="True" w786 {
              tunnel: [Commande_1."Sceaux 0" Commande_1."Sceaux 1"] -> w787
              tunnel: w783 -> [w789 w796]
              tunnel: [w788 w795] -> w782
              frame False {
                n208 = call "Sous_VI_acq_ligne.vi"("Seuil"=150, "error in (no error)"=w789) -> ("Décalage"=w793:u32, "G/D ?"=w791:bool, "error out"=w790:errorcluster)  [unwired: 8 in, 3 out]
                n209 = call "Sous_VI_correction.vi"("error in (no error)"=w790, "G/D ?"=w791, "Décalage"=w793) -> ("error out"=w788:errorcluster)  [unwired: 8 in]
              }
              frame True {
                n210 = while {
                  shift-right: [w798] -> w795
                  shift-left: w796 -> [w799]
                  i -> [w803]
                  stop <- w800 stop-if-true
                  n211 = Greater Or Equal?(x=w803, y=200) -> (x >= y?=w801:bool)
                  n212 = case shown="False" w801 {
                    tunnel: [FALSE TRUE] -> w800
                    tunnel: w799 -> [w805 w811]
                    tunnel: [w804 w811] -> w798
                    frame False {
                      n213 = call "Sous_VI_acq_ligne.vi"("Seuil"=150, "error in (no error)"=w805) -> ("Décalage"=w810:u32, "G/D ?"=w807:bool, "error out"=w806:errorcluster)  [unwired: 8 in, 3 out]
                      n214 = call "Sous_VI_correction.vi"("error in (no error)"=w806, "G/D ?"=w807, "Décalage"=w810) -> ("error out"=w804:errorcluster)  [unwired: 8 in]
                    }
                    frame True {
                    }
                  }
                }
              }
            }
          }
          frame "Sceaux 1" {
            # "Ignore le sceaux 1"
            n215 = case shown="False" w816 {
              tunnel: [T1 {"Bras"=TRUE, "Avance"=TRUE, "Tourne"=TRUE, "Sceaux"=FALSE, "Virage 2"=FALSE, "Trieur"=FALSE, "Bras 2"=FALSE, "Clapet 2"=FALSE, "Virage 3"=FALSE, "Virage 4"=FALSE, "Lanceur"=FALSE} ("Cluster 2") T1 {"Bras"=TRUE, "Avance"=TRUE, "Tourne"=TRUE, "Sceaux"=TRUE, "Virage 2"=TRUE, "Trieur"=TRUE, "Bras 2"=TRUE, "Clapet 2"=TRUE, "Virage 3"=TRUE, "Virage 4"=TRUE, "Lanceur"=TRUE} ("Cluster 2")] -> w817
              tunnel: [w822 w829] -> w814
              tunnel: w813 -> [w821 w828]
              frame False {
                n216 = call "Sous_VI_acq_ligne.vi"("Seuil"=150, "error in (no error)"=w821) -> ("Décalage"=w826:u32, "G/D ?"=w824:bool, "error out"=w823:errorcluster)  [unwired: 8 in, 3 out]
                n217 = call "Sous_VI_correction.vi"("error in (no error)"=w823, "G/D ?"=w824, "Décalage"=w826) -> ("error out"=w822:errorcluster)  [unwired: 8 in]
              }
              frame True {
                n218 = while {
                  shift-right: [w833] -> w829
                  shift-left: w828 -> [w834]
                  i -> [w839]
                  stop <- w835 stop-if-true
                  n219 = call "Sous_VI_acq_ligne.vi"("Seuil"=150, "error in (no error)"=w834) -> ("Décalage"=w836:u32, "G/D ?"=w831:bool, "error out"=w832:errorcluster)  [unwired: 8 in, 3 out]
                  n220 = Greater Or Equal?(x=w839, y=200) -> (x >= y?=w835:bool)
                  n221 = call "Sous_VI_correction.vi"("error in (no error)"=w832, "G/D ?"=w831, "Décalage"=w836) -> ("error out"=w833:errorcluster)  [unwired: 8 in]
                }
              }
            }
            n222 = Select(t=Commande_1."Sceaux 2", s=w816, f=Commande_1."Sceaux 1") -> (s? t:f=w818:T2)
          }
          frame "Sceaux 2" {
            # "Ignore le sceaux 2"
            n223 = case shown="True" w842 {
              tunnel: [T1 {"Bras"=TRUE, "Avance"=TRUE, "Tourne"=TRUE, "Sceaux"=FALSE, "Virage 2"=FALSE, "Trieur"=FALSE, "Bras 2"=FALSE, "Clapet 2"=FALSE, "Virage 3"=FALSE, "Virage 4"=FALSE, "Lanceur"=FALSE} ("Cluster 2") T1 {"Bras"=TRUE, "Avance"=TRUE, "Tourne"=TRUE, "Sceaux"=TRUE, "Virage 2"=TRUE, "Trieur"=TRUE, "Bras 2"=TRUE, "Clapet 2"=TRUE, "Virage 3"=TRUE, "Virage 4"=TRUE, "Lanceur"=TRUE} ("Cluster 2")] -> w843
              tunnel: [w849 w856] -> w840
              tunnel: w841 -> [w848 w855]
              frame False {
                n224 = call "Sous_VI_acq_ligne.vi"("Seuil"=150, "error in (no error)"=w848) -> ("Décalage"=w853:u32, "G/D ?"=w851:bool, "error out"=w850:errorcluster)  [unwired: 8 in, 3 out]
                n225 = call "Sous_VI_correction.vi"("error in (no error)"=w850, "G/D ?"=w851, "Décalage"=w853) -> ("error out"=w849:errorcluster)  [unwired: 8 in]
              }
              frame True {
                n226 = while {
                  shift-right: [w860] -> w856
                  shift-left: w855 -> [w861]
                  i -> [w866]
                  stop <- w862 stop-if-true
                  n227 = call "Sous_VI_acq_ligne.vi"("Seuil"=150, "error in (no error)"=w861) -> ("Décalage"=w863:u32, "G/D ?"=w858:bool, "error out"=w859:errorcluster)  [unwired: 8 in, 3 out]
                  n228 = Greater Or Equal?(x=w866, y=200) -> (x >= y?=w862:bool)
                  n229 = call "Sous_VI_correction.vi"("error in (no error)"=w859, "G/D ?"=w858, "Décalage"=w863) -> ("error out"=w860:errorcluster)  [unwired: 8 in]
                }
              }
            }
            n230 = Select(t=Commande_1."Sceaux 3", s=w842, f=Commande_1."Sceaux 2") -> (s? t:f=w845:T2)
          }
          frame "Sceaux 3" {
            # "Tapper la balle sur le sceau 3 avec le bras"
            n231 = case shown="False" w872 {
              tunnel: [T1 {"Bras"=TRUE, "Avance"=TRUE, "Tourne"=TRUE, "Sceaux"=FALSE, "Virage 2"=FALSE, "Trieur"=FALSE, "Bras 2"=FALSE, "Clapet 2"=FALSE, "Virage 3"=FALSE, "Virage 4"=FALSE, "Lanceur"=FALSE} ("Cluster 2") T1 {"Bras"=TRUE, "Avance"=TRUE, "Tourne"=TRUE, "Sceaux"=TRUE, "Virage 2"=TRUE, "Trieur"=TRUE, "Bras 2"=TRUE, "Clapet 2"=TRUE, "Virage 3"=TRUE, "Virage 4"=TRUE, "Lanceur"=TRUE} ("Cluster 2")] -> w871
              tunnel: [w876 w883] -> w868
              tunnel: w867 -> [w875 w882]
              frame False {
                n232 = call "Sous_VI_acq_ligne.vi"("Seuil"=150, "error in (no error)"=w875) -> ("Décalage"=w880:u32, "G/D ?"=w878:bool, "error out"=w877:errorcluster)  [unwired: 8 in, 3 out]
                n233 = call "Sous_VI_correction.vi"("error in (no error)"=w877, "G/D ?"=w878, "Décalage"=w880) -> ("error out"=w876:errorcluster)  [unwired: 8 in]
              }
              frame True {
                n234 = call "Sous_VI_Sceaux.vi"("error in (no error)"=w882) -> ("error out"=w883:errorcluster)  [unwired: 10 in]
              }
            }
            n235 = Select(t=Commande_1."Sceaux 4", s=w872, f=Commande_1."Sceaux 3") -> (s? t:f=w869:T2)
          }
          frame "Sceaux 4" {
            # "Tapper la balle sur le sceau 4 avec le bras"
            n236 = while {
              shift-right: [w896] -> w887
              shift-left: w885 -> [w897]
              i -> [w901]
              stop <- w898 stop-if-true
              n237 = Greater Or Equal?(x=w901, y=400) -> (x >= y?=w899:bool)
              n238 = case shown="False" w899 {
                tunnel: [FALSE TRUE] -> w898
                tunnel: w897 -> [w903 w909]
                tunnel: [w902 w909] -> w896
                frame False {
                  n239 = call "Sous_VI_acq_ligne.vi"("Seuil"=150, "error in (no error)"=w903) -> ("Décalage"=w907:u32, "G/D ?"=w904:bool, "error out"=w905:errorcluster)  [unwired: 8 in, 3 out]
                  n240 = call "Sous_VI_correction.vi"("error in (no error)"=w905, "G/D ?"=w904, "Décalage"=w907) -> ("error out"=w902:errorcluster)  [unwired: 8 in]
                }
                frame True {
                }
              }
            }
            n241 = call "Sous_VI_Sceaux.vi"("error in (no error)"=w887) -> ("error out"=w888:errorcluster)  [unwired: 10 in]
            n242 = call "Sous_VI_acq_ligne.vi"("Seuil"=150, "error in (no error)"=w888) -> ("Décalage"=w892:u32, "G/D ?"=w890:bool, "error out"=w889:errorcluster)  [unwired: 8 in, 3 out]
            n243 = call "Sous_VI_correction.vi"("error in (no error)"=w889, "G/D ?"=w890, "Décalage"=w892) -> ("error out"=w886:errorcluster)  [unwired: 8 in]
          }
          frame "Virage 2" {
            # "Effectuer le 2 eme virage"
            n244 = case shown="True" w914 {
              tunnel: [T1 {"Bras"=TRUE, "Avance"=TRUE, "Tourne"=TRUE, "Sceaux"=FALSE, "Virage 2"=FALSE, "Trieur"=FALSE, "Bras 2"=FALSE, "Clapet 2"=FALSE, "Virage 3"=FALSE, "Virage 4"=FALSE, "Lanceur"=FALSE} ("Cluster 2") T1 {"Bras"=TRUE, "Avance"=TRUE, "Tourne"=TRUE, "Sceaux"=TRUE, "Virage 2"=FALSE, "Trieur"=FALSE, "Bras 2"=FALSE, "Clapet 2"=FALSE, "Virage 3"=FALSE, "Virage 4"=FALSE, "Lanceur"=FALSE} ("Cluster 2")] -> w918
              tunnel: [w920 w927] -> w912
              tunnel: w911 -> [w919 w926]
              frame False {
                n245 = call "Sous_VI_acq_ligne.vi"("Seuil"=150, "error in (no error)"=w919) -> ("Décalage"=w924:u32, "G/D ?"=w922:bool, "error out"=w921:errorcluster)  [unwired: 8 in, 3 out]
                n246 = call "Sous_VI_correction.vi"("error in (no error)"=w921, "G/D ?"=w922, "Décalage"=w924) -> ("error out"=w920:errorcluster)  [unwired: 8 in]
              }
              frame True {
                n247 = call "Sous_VI_Virage_1.vi"("error in (no error)"=w926) -> ("error out"=w927:errorcluster)  [unwired: 10 in]
              }
            }
            n248 = Select(t=Commande_1."Recule", s=w914, f=Commande_1."Virage 2") -> (s? t:f=w915:T2)
          }
          frame "Recule" {
            # "Avance jusqu'à la ligne de gauche \npuis recule jusqu'à la zone de tri"
            n249 = case shown="False" w933 {
              tunnel: [Commande_1."Recule" Commande_1."Trieur"] -> w932
              tunnel: [w936 w943] -> w930
              tunnel: w929 -> [w935 w942]
              frame False {
                n250 = call "Sous_VI_acq_ligne.vi"("Seuil"=150, "error in (no error)"=w935) -> ("Décalage"=w939:u32, "G/D ?"=w938:bool, "error out"=w937:errorcluster)  [unwired: 8 in, 3 out]
                n251 = call "Sous_VI_correction.vi"("error in (no error)"=w937, "G/D ?"=w938, "Décalage"=w939) -> ("error out"=w936:errorcluster)  [unwired: 8 in]
              }
              frame True {
                n252 = call "Sous_VI_recule.vi"("error in (no error)"=w942) -> ("error out"=w943:errorcluster)  [unwired: 10 in]
              }
            }
          }
          frame "Trieur" {
            # "Effectue le tri des balle en fonction de leur couleur:\nfaire tomber les balles orange"
            n253 = while {
              shift-right: [w953] -> w947
              shift-left: w945 -> [w952]
              i -> [w957]
              stop <- w955 stop-if-true
              w954 = 0.0 ("moteur gauche vite")
              n254 = Less?(x=2000, y=w957) -> (x < y?=w955:bool)
              n255 = call "Sous_VI_moteurs.vi"("error in (no error)"=w952, "Moteur Droit"=w954, "Moteur Gauche"=w954) -> ("error out"=w953:errorcluster)  [unwired: 8 in]
            }
            n256 = call "Labview_trieur_balles.vi"("error in (no error)"=w947, "Numeric"=4) -> ("error out"=w946:errorcluster)  [unwired: 9 in]
          }
          frame "Intersection" {
            # "Ignore la 1 ere ligne a gauche"
            n257 = case shown="False" w960 {
              tunnel: w959 -> [w967 w973]
              tunnel: [w966 w972] -> w958
              frame False {
                n258 = call "Sous_VI_acq_ligne.vi"("Seuil"=150, "error in (no error)"=w967) -> ("Décalage"=w970:u32, "G/D ?"=w969:bool, "error out"=w968:errorcluster)  [unwired: 8 in, 3 out]
                n259 = call "Sous_VI_correction.vi"("error in (no error)"=w968, "G/D ?"=w969, "Décalage"=w970) -> ("error out"=w966:errorcluster)  [unwired: 8 in]
              }
              frame True {
                n260 = while {
                  shift-right: [w974] -> w972
                  shift-left: w973 -> [w975]
                  i -> [w982]
                  stop <- w978 stop-if-true
                  n261 = call "Sous_VI_acq_ligne.vi"("Seuil"=150, "error in (no error)"=w975) -> ("Décalage"=w979:u32, "G/D ?"=w977:bool, "error out"=w976:errorcluster)  [unwired: 8 in, 3 out]
                  n262 = Greater Or Equal?(x=w982, y=200) -> (x >= y?=w978:bool)
                  n263 = call "Sous_VI_correction.vi"("error in (no error)"=w976, "G/D ?"=w977, "Décalage"=w979) -> ("error out"=w974:errorcluster)  [unwired: 8 in]
                }
              }
            }
            n264 = Select(t=Commande_1."Intersection4", s=w960, f=Commande_1."Intersection") -> (s? t:f=w963:T2)
          }
          frame "Intersection4" {
            # "Ignore la 2 eme ligne a gauche"
            n265 = call "Sous_VI_acq_ligne.vi"("Seuil"=150, "error in (no error)"=w983) -> ("Décalage"=w987:u32, "G/D ?"=w986:bool, "error out"=w985:errorcluster)  [unwired: 8 in, 3 out]
            n266 = call "Sous_VI_correction.vi"("error in (no error)"=w985, "G/D ?"=w986, "Décalage"=w987) -> ("error out"=w984:errorcluster)  [unwired: 8 in]
            n267 = Select(t=Commande_1."Bras 2", s=w991, f=Commande_1."Intersection4") -> (s? t:f=w990:T2)
          }
          frame "Bras 2" {
            w998 = 0.0 ("moteur gauche vite")
            # "Bras en position pour les clapets"
            n268 = while {
              shift-right: [w1005] -> w997
              shift-left: w995 -> [w1004]
              i -> [w1012]
              stop <- w1010 stop-if-true
              n269 = call "Sous_VI_acq_ligne.vi"("Seuil"=150, "error in (no error)"=w1004) -> ("Décalage"=w1008:u32, "G/D ?"=w1007:bool, "error out"=w1006:errorcluster)  [unwired: 8 in, 3 out]
              n270 = Less?(x=1500, y=w1012) -> (x < y?=w1010:bool)
              n271 = call "Sous_VI_correction.vi"("error in (no error)"=w1006, "G/D ?"=w1007, "Décalage"=w1008) -> ("error out"=w1005:errorcluster)  [unwired: 8 in]
            }
            n272 = call "Sous_VI_moteurs.vi"("error in (no error)"=w997, "Moteur Droit"=w998, "Moteur Gauche"=w998) -> ("error out"=w999:errorcluster)  [unwired: 8 in]
            n273 = call "Sous_VI_Bras.vi"("error in (no error)"=w999, "Enum bras"=enum_bras."Clapet Bras") -> ("error out"=w996:errorcluster)  [unwired: 9 in]
          }
          frame "Clapet 2" {
            # "Avance en faisant tomber les clapets avec le bras"
            n274 = call "Sous_VI_acq_ligne.vi"("Seuil"=150, "error in (no error)"=w1013) -> ("Décalage"=w1023:u32, "G/D ?"=w1016:bool, "error out"=w1015:errorcluster)  [unwired: 8 in, 3 out]
            n275 = call "Sous_VI_correction.vi"("error in (no error)"=w1015, "G/D ?"=w1016, "Décalage"=w1023) -> ("error out"=w1014:errorcluster)  [unwired: 8 in]
            n276 = Select(t=Commande_1."Virage 3", s=w1017, f=Commande_1."Clapet 2") -> (s? t:f=w1019:T2)
          }
          frame "Virage 3" {
            # "Effectuer le 3 eme virage"
            n277 = while {
              shift-right: [w1044] -> w1027
              shift-left: w1028 -> [w1045]
              i -> [w1048]
              stop <- w1047 stop-if-true
              w1046 = 0.0 ("moteur gauche vite")
              n278 = Less?(x=1000, y=w1048) -> (x < y?=w1047:bool)
              n279 = call "Sous_VI_moteurs.vi"("error in (no error)"=w1045, "Moteur Droit"=w1046, "Moteur Gauche"=w1046) -> ("error out"=w1044:errorcluster)  [unwired: 8 in]
            }
            n280 = while {
              shift-right: [w1032] -> w1026
              shift-left: w1027 -> [w1033]
              i -> [w1034]
              stop <- w1036 stop-if-true
              n281 = Greater Or Equal?(x=w1034, y=100000) -> (x >= y?=w1037:bool)
              n282 = case shown="True" w1037 {
                tunnel: [FALSE TRUE] -> w1036
                tunnel: w1033 -> [w1039 w1042]
                tunnel: [w1038 w1042] -> w1032
                frame False {
                  n283 = call "Sous_VI_Bras.vi"("error in (no error)"=w1039, "Enum bras"=enum_bras."Inactif Bras") -> ("error out"=w1038:errorcluster)  [unwired: 9 in]
                }
                frame True {
                }
              }
            }
            n284 = call "Sous_VI_Virage_1.vi"("error in (no error)"=w1026) -> ("error out"=w1025:errorcluster)  [unwired: 10 in]
          }
          frame "Avance" {
            # "Avance jusqu'a la prochaine ligne à droite"
            n285 = call "Sous_VI_acq_ligne.vi"("Seuil"=150, "error in (no error)"=w1050) -> ("Décalage"=w1056:u32, "G/D ?"=w1053:bool, "error out"=w1052:errorcluster)  [unwired: 8 in, 3 out]
            n286 = call "Sous_VI_correction.vi"("error in (no error)"=w1052, "G/D ?"=w1053, "Décalage"=w1056) -> ("error out"=w1051:errorcluster)  [unwired: 8 in]
            n287 = Select(t=Commande_1."Virage 4", s=w1057, f=Commande_1."Avance") -> (s? t:f=w1058:T2)
          }
          frame "Virage 4" {
            # "Effectuer le 4 eme virage"
            n288 = call "Sous_VI_Virage_1.vi"("error in (no error)"=w1062) -> ("error out"=w1063:errorcluster)  [unwired: 10 in]
          }
          frame "Lanceur" {
            # "Se place en position devant la cible, met en route le moteur\nde la roue qui lance les balles puis le moteur du distributeur\npour lancer les balles sur la cible \nEteint les moteur"
            n289 = call "Sous_VI_Lanceur.vi"("error in (no error)"=w1067, "Nb balles"=2) -> ("error out"=w1068:errorcluster)  [unwired: 9 in]
          }
          frame "Demi_tour" {
            # "Faire demi tour"
            n290 = call "Sous_VI_Virage_1.vi"("error in (no error)"=w1073) -> ("error out"=w1074:errorcluster)  [unwired: 10 in]
          }
          frame "Virage 5" {
            # "Effectuer le 5 eme virage"
            n291 = case shown="False" w1082 {
              tunnel: [Commande_1."Virage 5" Commande_1."Virage 6"] -> w1083
              tunnel: [w1085 w1092] -> w1079
              tunnel: w1078 -> [w1084 w1091]
              frame False {
                n292 = call "Sous_VI_acq_ligne.vi"("Seuil"=150, "error in (no error)"=w1084) -> ("Décalage"=w1090:u32, "G/D ?"=w1087:bool, "error out"=w1086:errorcluster)  [unwired: 8 in, 3 out]
                n293 = call "Sous_VI_correction.vi"("error in (no error)"=w1086, "G/D ?"=w1087, "Décalage"=w1090) -> ("error out"=w1085:errorcluster)  [unwired: 8 in]
              }
              frame True {
                n294 = call "Sous_VI_Virage_cible.vi"("error in (no error)"=w1091) -> ("error out"=w1092:errorcluster)  [unwired: 10 in]
              }
            }
          }
          frame "Virage 6" {
            # "Effectuer le 6 eme virage"
            n295 = case shown="True" w1099 {
              tunnel: [Commande_1."Virage 6" Commande_1."End"] -> w1098
              tunnel: [w1101 w1108] -> w1095
              tunnel: w1094 -> [w1100 w1107]
              frame False {
                n296 = call "Sous_VI_acq_ligne.vi"("Seuil"=150, "error in (no error)"=w1100) -> ("Décalage"=w1106:u32, "G/D ?"=w1103:bool, "error out"=w1102:errorcluster)  [unwired: 8 in, 3 out]
                n297 = call "Sous_VI_correction.vi"("error in (no error)"=w1102, "G/D ?"=w1103, "Décalage"=w1106) -> ("error out"=w1101:errorcluster)  [unwired: 8 in]
              }
              frame True {
                n298 = call "Sous_VI_Virage_1.vi"("error in (no error)"=w1107) -> ("error out"=w1108:errorcluster)  [unwired: 10 in]
              }
            }
          }
          frame "End" {
            w1112 = 0.0 ("moteur gauche vite")
            # "Fin du programme"
            n299 = call "Sous_VI_moteurs.vi"("error in (no error)"=w1111, "Moteur Droit"=w1112, "Moteur Gauche"=w1112) -> ("error out"=w1110:errorcluster)  [unwired: 8 in]
          }
        }
      }
    }
    "Cluster 3" <- w28
    "Énum 2" <- w34
    n300 = node-c288(w9) -> ()  [unwired: 1 out]
  }
  n301 = node-c288(w6) -> (→"error out":errorcluster)
